vi "Configuration Utility.vi"() -> ()   [LabVIEW 2014, in "Standard Editor.lvlib"]
doc: "This is the main VI for the configuration editor."
uses:
  Standard Editor.lvlib
  Controls/StateCluster.ctl
  Configuration Editor/Classes/SystemConfigRepo/SystemConfigRepo.lvclass
  Configuration Editor/Classes/Systems/Systems.lvclass
  <vilib>/NI/Configuration Framework/Node/StandardEvents.ctl
  <vilib>/NI/Configuration Framework/Node/UserEventRef.ctl
  <vilib>/NI/Configuration Framework/Controls/EventCluster.ctl
  <vilib>/NI/Configuration Framework/Node/NodeChangeEvent.ctl
  <vilib>/NI/Configuration Framework/Node/NodeRef.ctl
  <vilib>/NI/Configuration Framework/Node/NISE_CEF_Node.lvclass
  <vilib>/NI/Configuration Framework/Node/CacheState.ctl
  <vilib>/NI/Configuration Framework/Node/RefreshUIEvent.ctl
  <vilib>/NI/Configuration Framework/Node/StopEvent.ctl
  <vilib>/NI/Configuration Framework/glyph manager/glyph manager.ctl
  <vilib>/picture/picture.llb/imagedata.ctl
  <vilib>/NI/AMC/Message Queue.ctl
  <vilib>/NI/AMC/Message.ctl
  <vilib>/NI/Tools/Keyed Array/KeyedArray.ctl
  Controls/add message.ctl
  Controls/MoveMessage.ctl
  <vilib>/NI/Progress Bar/Controls/Progress Bar Properties.ctl
  <vilib>/NI/Progress Bar/Controls/Update Bar Actions.ctl
  <vilib>/NI/AMC/Create Single Message.vi
  <vilib>/NI/AMC/Update Message Routing Info.vi
  <vilib>/NI/AMC/Read Termination Message.vi
  Configuration Editor/subVIs/Glyphs Status.ctl
  Configuration Editor/subVIs/Add status to name.vi
  <vilib>/NI/AMC/Send Message.vi
  <vilib>/NI/AMC/Globals.vi
  Configuration Editor/Classes/Module editor node/module editor node.lvclass
  Configuration Editor/Classes/EngineTags/EngineTags.lvclass
  <vilib>/NI/Module Timing Source/timing source/TBM timing source.lvclass
  Configuration Editor/Classes/TBM Configuration Node/TBM Configuration Node.lvclass
  <vilib>/NI/Tag Bus Module Framework/root configuration/TBM configuration.lvclass
  Framework Configuration Classes/target configuration/PL_Target Configuration.lvclass
  Configuration Editor/Classes/Targets/Targets.lvclass
  Configuration Editor/Classes/Engine Parent/Engine Parent Editor Node.lvclass
  <vilib>/NI/Configuration Framework/Repository/NISE_CEF_Repository.lvclass
  Framework Configuration Classes/system configuration/PL_System Configuration.lvclass
  <vilib>/NI/Module Execution Interface/Engine Configuration/engine configuration.lvclass
  <vilib>/NI/Tag Bus Module Framework/channel/TBM channel.lvclass
  <vilib>/NI/Tag Bus Module Framework/module configuration/TBM module configuration.lvclass
  <vilib>/NI/AMC/AMC.lvlib
  <vilib>/NI/Configuration Framework/NISE_CEF_TreeControl.lvlib
  Framework Configuration Classes/class cache/PL_class cache.lvlib
  Configuration Editor/PL Framework Configuration Tool.lvlib
  <vilib>/NI/Configuration Framework/hierarchy repo/NISE_CEF_HierarchyRepo.lvclass
  <vilib>/NI/Configuration Framework/tree serializer/NISE_CEF_TreeSerializer.lvlib
  <vilib>/NI/Configuration Framework/glyph manager/glyph manager.lvlib
  <vilib>/NI/Tools/Keyed Array/Tools_KeyedArray.lvlib
  <vilib>/NI/Progress Bar/Progress Bar.lvlib
  about menu/About Screen Library.lvlib
  INI Configuration/DCAF INI.lvlib
panel:
  in  "Exit":bool
  in  "View":string(tree)
  # "DCAF Editor"
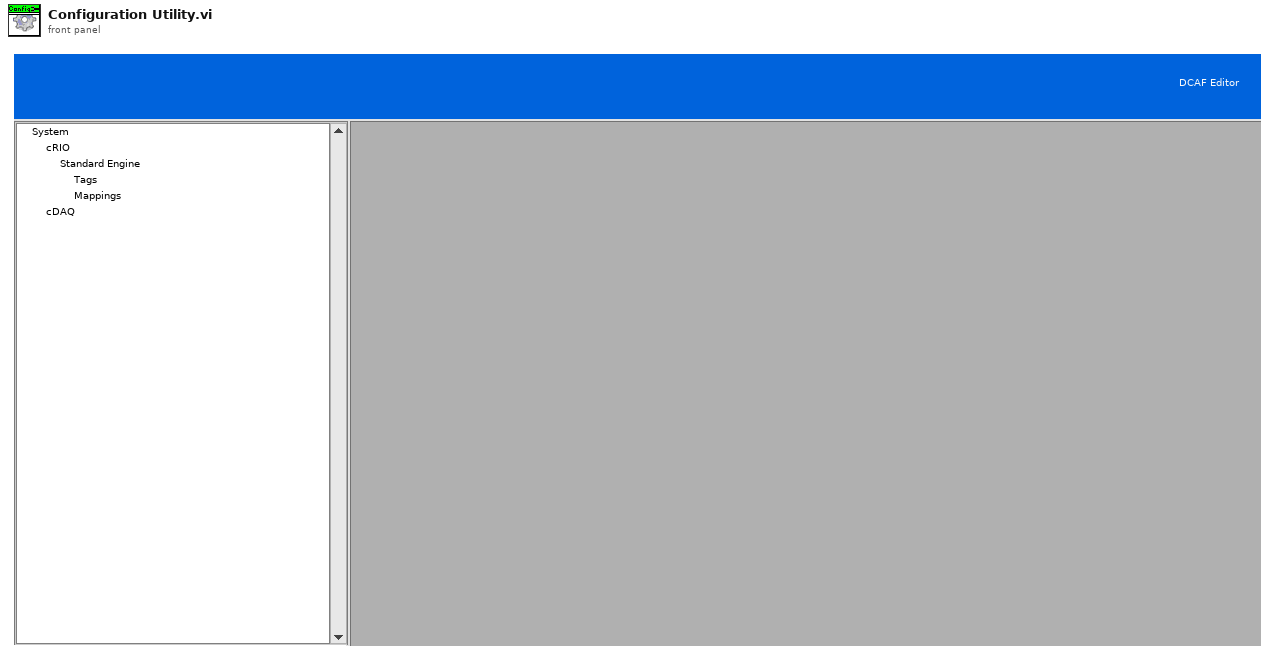
[diagram p1: front panel]
types:
  T1 = enum32{"Invalid", "Standard", "Closed", "Hidden", "Minimized", "Maximized"}
  T2 = typedef "Standard Editor.lvlib/StateCluster.ctl" = cluster{"repository":refnum<class "SystemConfigRepo.lvclass">, "root":refnum<data-value>, "unsaved changes":bool, "current path":path, "classes cache":path, "standard events":T3, "glyph manager":T9, "VI ref":refnum<vi>, "main queue":T11, "Sub Panel":refnum<vi>}
  T3 = typedef "NISE_CEF_Node.lvclass/StandardEvents.ctl" = cluster{"user event":T4, "node change":T5, "cache state":T6, "refresh UI":T7, "stop event":T8}
  T4 = typedef "NISE_CEF_Node.lvclass/UserEventRef.ctl" = refnum<user-event>
  T5 = typedef "NISE_CEF_Node.lvclass/NodeChangeEvent.ctl" = refnum<user-event>
  T6 = typedef "NISE_CEF_Node.lvclass/CacheState.ctl" = refnum<user-event>
  T7 = typedef "NISE_CEF_Node.lvclass/RefreshUIEvent.ctl" = refnum<user-event>
  T8 = typedef "NISE_CEF_Node.lvclass/StopEvent.ctl" = refnum<user-event>
  T9 = typedef "glyph manager.lvlib/glyph manager.ctl" = cluster{"search paths":path[], "glyph map":variant, "base glyphs":T10[], "desired overlays":string[]}
  T10 = typedef "imagedata.ctl" = cluster{"image type":i32, "image depth":i32, "image":u8[], "mask":u8[], "colors":u32[], "Rectangle":cluster{"left":i16, "top":i16, "right":i16, "bottom":i16}}
  T11 = typedef "AMC.lvlib/Message Queue.ctl" = refnum<queue>
  T12 = cluster{"node id":string, "RightClickPath":string}
  T13 = typedef "Standard Editor.lvlib/add message.ctl" = cluster{"node type":string, "to add to":string}
  T14 = typedef "Standard Editor.lvlib/MoveMessage.ctl" = cluster{"node ref":T15, "new parent":T15, "Index":i32}
  T15 = typedef "NISE_CEF_Node.lvclass/NodeRef.ctl" = refnum<data-value>
  T16 = typedef "LVPoint32TypeDef.ctl" = cluster{"Horizontal":i32, "Vertical":i32}
  T17 = cluster{"data name":string, "drag data":variant}[]
  T18 = typedef "NISE_CEF_Node.lvclass/NodeMenuOptions.ctl" = cluster{"removable":bool, "movable":bool, "duplicate":bool}
  T19 = typedef "Progress Bar.lvlib/Progress Bar Properties.ctl" = cluster{"Background Color":u32, "Installer Title":string, "Title Color":u32, "Action Text":string, "Text Color":u32, "Slider Value":u8, "Bar Color":u32, "Timeout":i32}
  T20 = typedef "Progress Bar.lvlib/Update Bar Actions.ctl" = enum16{"Add To Existing", "Set to Value"}
  T21 = typedef "Standard Editor.lvlib/FilePaths.ctl" = cluster{"glyphs":path[], "classes":path, "classes cache":path}
  T22 = typedef "PL_class cache.lvlib/cache definition.ctl" = cluster{"configuration":T23, "class cache data":T24}
  T23 = typedef "PL_class cache.lvlib/cache search configuration.ctl" = cluster{"Search Paths":path[], "Folders to Exclude":string[], "full class list":path[]}
  T24 = typedef "PL_class cache.lvlib/cached class information.ctl" = cluster{"targets":T25[], "engines":T26[], "modules":T26[], "ignored class list":path[]}
  T25 = typedef "PL_class cache.lvlib/target class metadata.ctl" = cluster{"file name":string, "fully qualified name":string, "menu display name":string, "configuration class name":string}
  T26 = typedef "PL_class cache.lvlib/class metadata.ctl" = cluster{"file name":string, "fully qualified name":string, "menu display name":string, "configuration class":string, "category":string, "instances allowed":i32, "supported targets":T27[]}
  T27 = typedef "TBM configuration.lvclass/Target Types.ctl" = enum16{"Windows", "Mac", "Linux", "Linux RT ARM", "VxWorks", "Pharlap", "Other", "Linux RT x64"}
  T28 = typedef "NISE_CEF_Node.lvclass/Summary.ctl" = cluster{"ID":string, "parent ID":string, "node type":string, "text":string, "additional text":string, "glyph":string, "depth":i32, "glyph overlay":string}
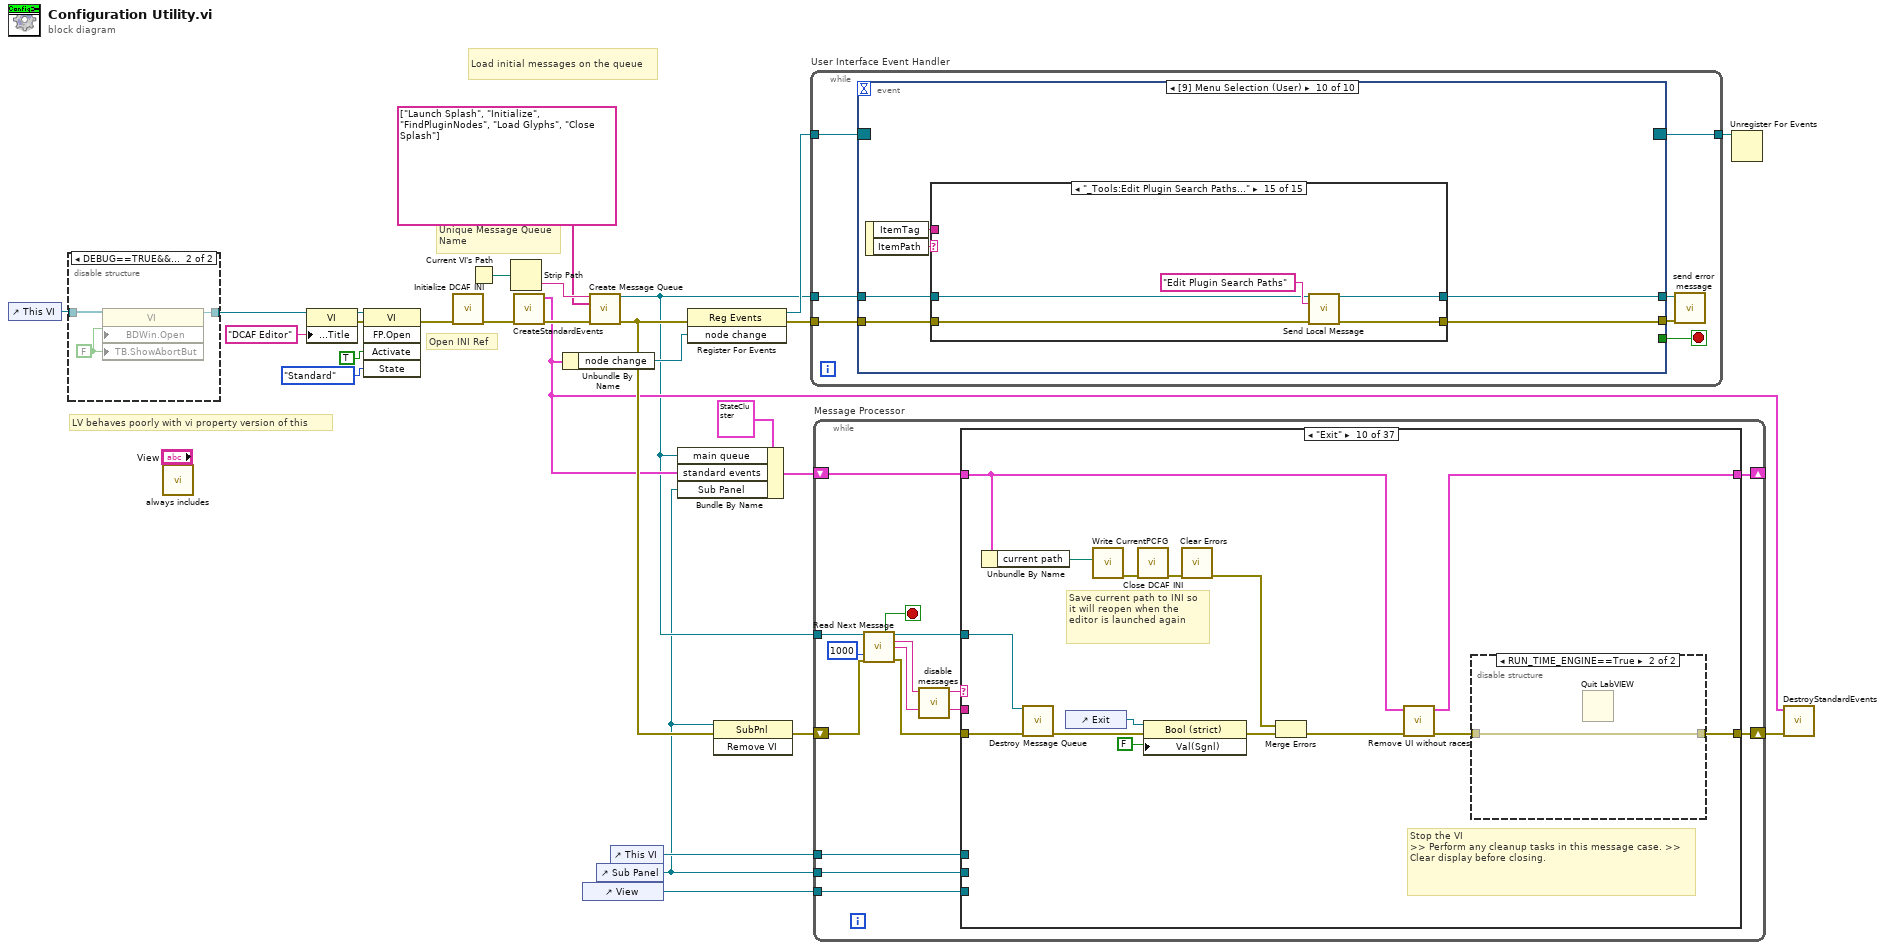
[diagram p0: block diagram]
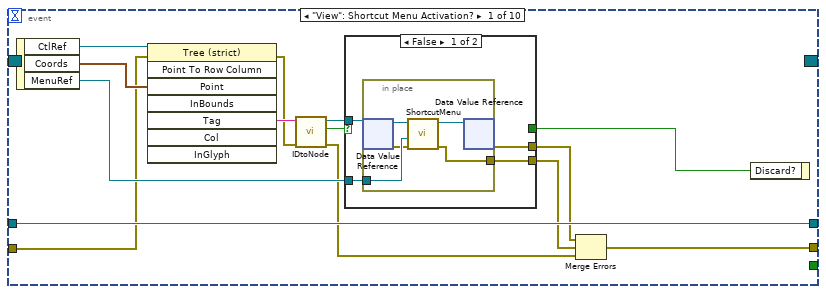
[diagram p3: hidden frame]
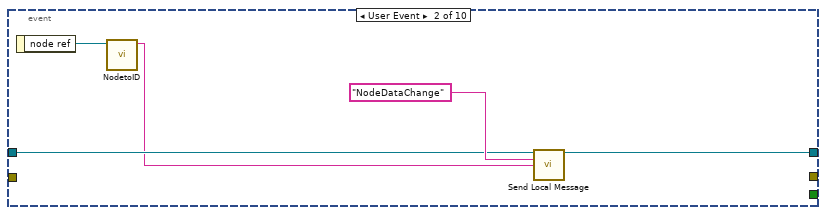
[diagram p5: hidden frame]
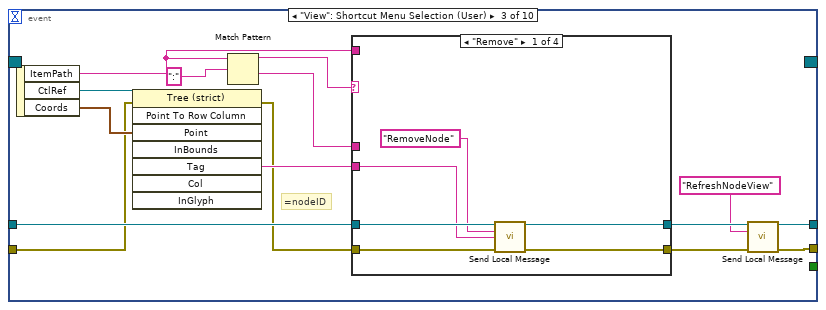
[diagram p6: hidden frame]
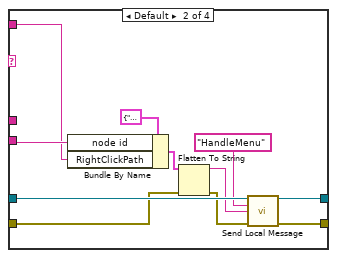
[diagram p7: hidden frame]
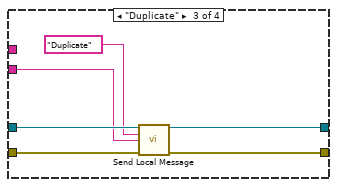
[diagram p8: hidden frame]
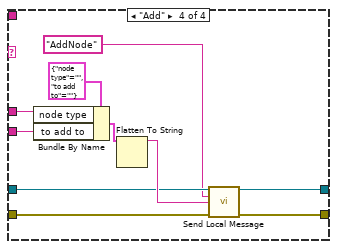
[diagram p9: hidden frame]
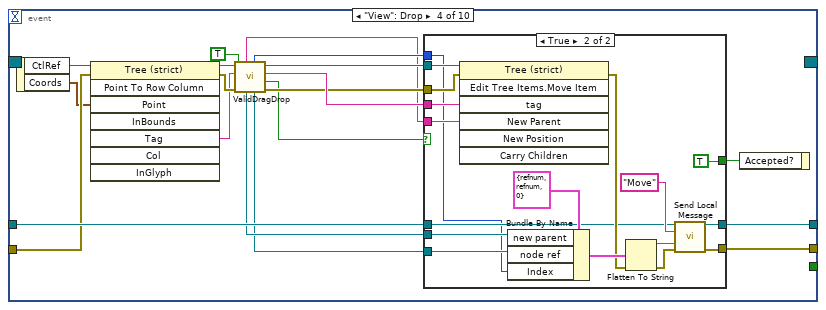
[diagram p10: hidden frame]
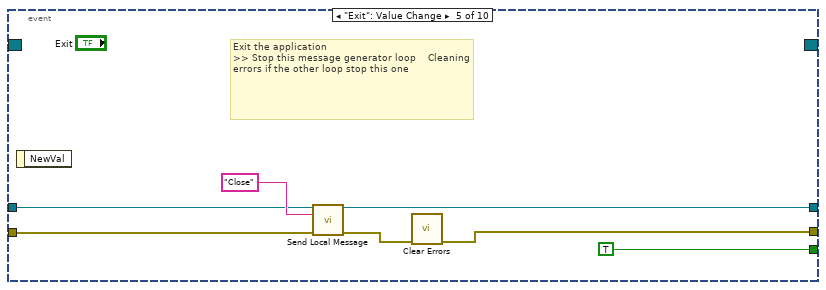
[diagram p12: hidden frame]
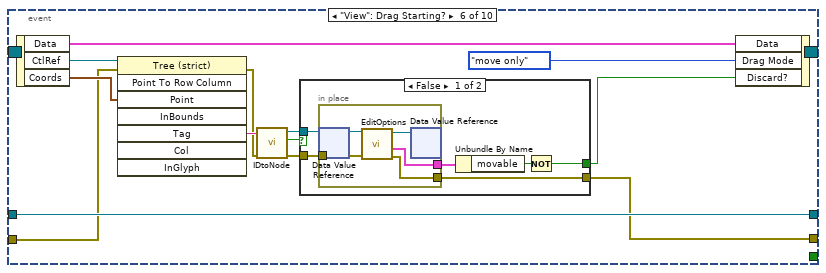
[diagram p13: hidden frame]
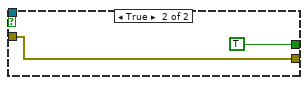
[diagram p14: hidden frame]
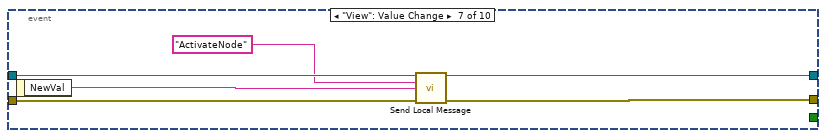
[diagram p15: hidden frame]
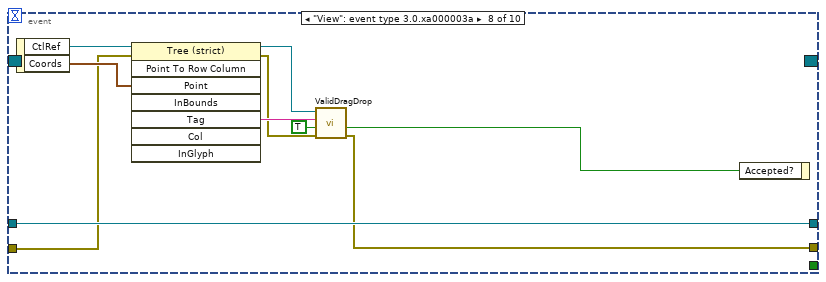
[diagram p16: hidden frame]
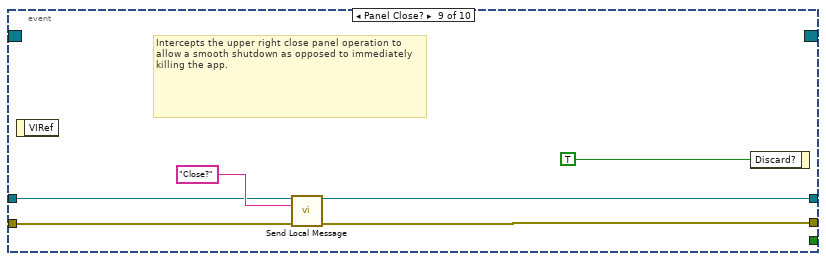
[diagram p17: hidden frame]
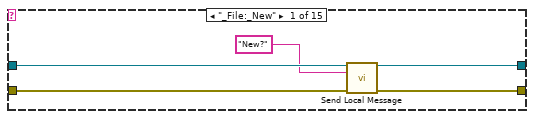
[diagram p18: hidden frame]
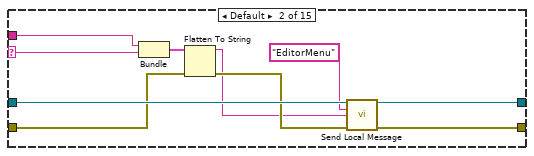
[diagram p19: hidden frame]
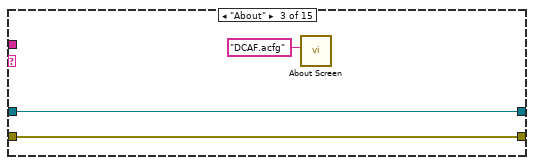
[diagram p20: hidden frame]
diagram:
  # "Open INI Ref"
  # "LV behaves poorly with vi property version of this"
  # "Unique Message Queue Name"
  # "Load initial messages on the queue"
  n1 = control-ref of="This VI"() -> (w20:refnum<vi>)
  n2 = disable-structure shown="DEBUG==TRUE&&RUN_TIME_ENGINE==False" {
    disable-tunnel: [w28 w31] -> w5
    disable-tunnel: w20 -> [w28 w30]
    frame condition #0 (active) {
    }
    frame condition #1 {
      w29 = FALSE ("Block Diagram Window:Open")
      n3 = property class="VI"(reference=w30, "BDWin.Open"=w29, "TB.ShowAbortBut"=w29) -> (reference out=w31:refnum<vi>)  [unwired: 1 in, 1 out]
    }
  }
  n4 = call "always includes.vi"() -> ()  [unwired: 12 in]
  n5 = property class="VI"(reference=w5, "Front Panel.Title"="DCAF Editor" ("Front Panel Window:Title")) -> (reference out=w4:refnum<vi>, error out=w6:errorcluster)  [unwired: 1 in]
  n6 = invoke class="VI" method="FP.Open"(reference=w4, error in=w6, "Activate"=TRUE ("Activate?"), "State"=T1."Standard") -> (error out=w1:errorcluster)  [unwired: 1 in, 4 out]
  n7 = call "Initialize DCAF INI.vi"("Error In"=w1) -> ("Error Out"=w2:errorcluster)  [unwired: 10 in]
  n8 = Current VI's Path() -> (path=w26:path)
  n9 = Strip Path(path=w26) -> (name=w27:string)  [unwired: 1 out]
  n10 = call <vilib>:"CreateStandardEvents.vi"("error in"=w2) -> ("error out"=w16:errorcluster, "standard events"=w9:T3)  [unwired: 9 in]
  n11 = Unbundle By Name(w9) -> ("node change"=w14:T5)
  n12 = control-ref of="View"() -> (w19:refnum<vi>)
  n13 = call <vilib>:"Create Message Queue.vi"("message queue name"=w27, "initial message names"=string[] ["Launch Splash", "Initialize", "FindPluginNodes", "Load Glyphs", "Close Splash"], "error in"=w16) -> ("message queue out"=w8:T11, "error out"=w23:errorcluster)  [unwired: 11 in]
  n14 = control-ref of="Sub Panel"() -> (w7:refnum<vi>)
  n15 = control-ref of="This VI"() -> (w17:refnum<vi>)
  n16 = Bundle By Name(cluster=T2 {"repository"=refnum, "root"=refnum, "unsaved changes"=FALSE, "current path"=path "", "classes cache"=path "", "standard events"={"user event"=refnum, "node change"=refnum, "cache state"=refnum, "refresh UI"=refnum, "stop event"=refnum}, "glyph manager"={"search paths"=[], "glyph map"=variant, "base glyphs"=[], "desired overlays"=[]}, "VI ref"=refnum, "main queue"=refnum, "Sub Panel"=refnum}, "main queue"=w8, "standard events"=w9, "Sub Panel"=w7) -> (w12:T2)
  n17 = register-events(error in=w23, w14) -> (reference out=w13:refnum<event-registration>, error out=w15:errorcluster)  [unwired: 1 in]
  n18 = invoke class="SubPnl" method="Remove VI"(reference=w7, error in=w23) -> (error out=w18:errorcluster)  [unwired: 1 in, 2 out]
  n19 = while "User Interface Event Handler" {
    tunnel: w8 -> [w38]
    tunnel: w15 -> [w34]
    tunnel: w13 -> [w33]
    tunnel: [w32] -> w11
    stop <- w37 stop-if-true
    n20 = event shown="[9] Menu Selection (User)" {
      selector: w33 -> [_ _ _ _ _ _ _ _ _ _]
      dyn-events: [_ _ _ _ _ _ _ _ _ _] -> w32
      timeout: _ -> [_ _ _ _ _ _ _ _ _ _]
      tunnel: w38 -> [w46 w65 w77 w125 w158 w165 w192 w197 w207 w213]
      tunnel: [_ _ _ _ TRUE _ _ _ _ _] -> w37
      tunnel: [w46 w64 w69 w127 w154 w165 w189 w197 w205 w212] -> w36
      tunnel: [w41 _ w70 w126 w155 w161 w188 w194 w203 w210] -> w35
      tunnel: w34 -> [w45 _ w75 w124 w156 w164 w187 w196 w204 w211]
      event "View": Shortcut Menu Activation? {
        n21 = event-data() -> ("CtlRef"=w52:refnum<vi>, "Coords"=w51:T16, "MenuRef"=w48:refnum<k9>)  [unwired: 1 in]
        n22 = invoke class="Tree (strict)" method="Point To Row Column"(reference=w52, error in=w45, "Point"=w51) -> (error out=w44:errorcluster, "Tag"=w50:string)  [unwired: 5 in, 6 out]
        n23 = call <vilib>:"IDtoNode.vi"("error in"=w44, "ID"=w50) -> ("error out"=w42:errorcluster, "invalid Id"=w47:bool, "node ref"=w49:T15)  [unwired: 7 in]
        n24 = case shown="False" w47 {
          selector: w47 -> [_ w62]
          tunnel: w49 -> [w56 _]
          tunnel: w48 -> [w55 _]
          tunnel: [w54 _] -> w43
          tunnel: [w53 _] -> w40
          tunnel: [_ w62] -> w39
          frame False {
            n25 = in-place {
              in-place-border: w55 -> [w59]
              in-place-border: [w57] -> w54
              n26 = in-place-dvr #1(w56) -> (w61:refnum<class "NISE_CEF_Node.lvclass">, w58:errorcluster)
              n27 = call-dynamic "ShortcutMenu.vi"("error in"=w58, "menu ref in"=w59, "node in"=w61) -> ("error out"=w57:errorcluster, "node out"=w60:refnum<class "NISE_CEF_Node.lvclass">)  [unwired: 6 in, 1 out]
              n28 = in-place-dvr #1(w60) -> (w53:errorcluster)  [unwired: 1 out]
            }
          }
          frame True {
          }
        }
        n29 = Merge Errors(w40, w43, w42) -> (w41:errorcluster)
        n30 = event-data("Discard?"=w39) -> ()  [unwired: 1 in, 1 out]
      }
      event User Event {
        n31 = event-data() -> ("node ref"=w67:T15)  [unwired: 1 in]
        n32 = call <vilib>:"NodetoID.vi"("node ref"=w67) -> ("ID"=w63:string)  [unwired: 9 in, 1 out]
        n33 = call <vilib>:"Send Local Message.vi"("message queue in"=w65, "message name"="NodeDataChange", "message value"=w63) -> ("message queue out"=w64:T11)  [unwired: 10 in, 2 out]
      }
      event "View": Shortcut Menu Selection (User) {
        # "=nodeID"
        n34 = event-data() -> ("ItemPath"=w73:string, "CtlRef"=w80:refnum<vi>, "Coords"=w81:T16)  [unwired: 1 in]
        n35 = invoke class="Tree (strict)" method="Point To Row Column"(reference=w80, error in=w75, "Point"=w81) -> (error out=w74:errorcluster, "Tag"=w76:string)  [unwired: 5 in, 6 out]
        n36 = Match Pattern(string=w73, regular expression=":") -> (before substring=w79:string, after substring=w78:string)  [unwired: 1 in, 2 out]
        n37 = case shown="\"Remove\"" w79 {
          tunnel: w78 -> [_ _ _ w110]
          tunnel: w77 -> [w88 w99 w105 w112]
          tunnel: w76 -> [w86 w93 w103 w111]
          tunnel: [w85 w97 w102 w108] -> w72
          tunnel: [w84 w96 w100 w106] -> w71
          tunnel: w74 -> [w83 w92 w101 w107]
          tunnel: w73 -> [_ w89 _ _]
          frame "Remove" {
            n38 = call <vilib>:"Send Local Message.vi"("message queue in"=w88, "message name"="RemoveNode" ("Message Name"), "message value"=w86, "error in"=w83) -> ("message queue out"=w85:T11, "error out"=w84:errorcluster)  [unwired: 9 in, 1 out]
          }
          frame Default {
            n39 = Bundle By Name(cluster=T12 {"node id"="", "RightClickPath"=""} ("input cluster"), "node id"=w93, "RightClickPath"=w89) -> (w94:T12)
            n40 = Flatten To String(anything=w94, error in (no error)=w92) -> (data string=w90:string, error out=w91:errorcluster)  [unwired: 2 in, 1 out]
            n41 = call <vilib>:"Send Local Message.vi"("message queue in"=w99, "message name"="HandleMenu" ("Message Name"), "message value"=w90, "error in"=w91) -> ("message queue out"=w97:T11, "error out"=w96:errorcluster)  [unwired: 9 in, 1 out]
          }
          frame "Duplicate" {
            n42 = call <vilib>:"Send Local Message.vi"("message queue in"=w105, "message name"="Duplicate" ("Message Name"), "message value"=w103, "error in"=w101) -> ("message queue out"=w102:T11, "error out"=w100:errorcluster)  [unwired: 9 in, 1 out]
          }
          frame "Add" {
            n43 = Bundle By Name(cluster=T13 {"node type"="", "to add to"=""} ("input cluster"), "node type"=w110, "to add to"=w111) -> (w113:T13)
            n44 = Flatten To String(anything=w113) -> (data string=w114:string)  [unwired: 3 in, 2 out]
            n45 = call <vilib>:"Send Local Message.vi"("message queue in"=w112, "message name"="AddNode" ("Message Name"), "message value"=w114, "error in"=w107) -> ("message queue out"=w108:T11, "error out"=w106:errorcluster)  [unwired: 9 in, 1 out]
          }
        }
        n46 = call <vilib>:"Send Local Message.vi"("message queue in"=w72, "message name"="RefreshNodeView", "error in"=w71) -> ("message queue out"=w69:T11, "error out"=w70:errorcluster)  [unwired: 10 in, 1 out]
      }
      event "View": Drop {
        n47 = event-data() -> ("CtlRef"=w123:refnum<vi>, "Coords"=w122:T16)  [unwired: 1 in]
        n48 = invoke class="Tree (strict)" method="Point To Row Column"(reference=w123, error in=w124, "Point"=w122) -> (reference out=w133:refnum<vi>, error out=w132:errorcluster, "Tag"=w130:string)  [unwired: 5 in, 5 out]
        n49 = call <vilib>:"ValidDragDrop.vi"("error in"=w132, "Reorder"=TRUE, "drag over"=w130, "Tree Ref in"=w133) -> ("Error Out"=w129:errorcluster, "Accepted"=w116:bool, "Drag"=w131:string, "Tree Ref out"=w134:refnum<vi>, "Moved Node"=w120:T15, "Position"=w119:i32, "Parent Node"=w121:T15, "Parent"=w118:string)
        n50 = case shown="True" w116 {
          tunnel: w131 -> [_ w151]
          tunnel: w134 -> [_ w153]
          tunnel: [_ TRUE] -> w128
          tunnel: w118 -> [_ w149]
          tunnel: w125 -> [w136 w138]
          tunnel: [w136 w145] -> w127
          tunnel: [w135 w144] -> w126
          tunnel: w120 -> [_ w140]
          tunnel: w121 -> [_ w139]
          tunnel: w129 -> [w135 w141]
          tunnel: w119 -> [_ w137]
          frame False {
          }
          frame True {
            n51 = invoke class="Tree (strict)" method="Edit Tree Items.Move Item"(reference=w153, error in=w141, "tag"=w151, "New Parent"=w149) -> (error out=w142:errorcluster)  [unwired: 3 in, 6 out]
            n52 = Bundle By Name(cluster=T14 {"node ref"=refnum, "new parent"=refnum, "Index"=0} ("Cluster"), "new parent"=w139, "node ref"=w140, "Index"=w137) -> (w148:T14)
            n53 = Flatten To String(anything=w148, error in (no error)=w142) -> (data string=w147:string, error out=w143:errorcluster)  [unwired: 2 in, 1 out]
            n54 = call <vilib>:"Send Local Message.vi"("message queue in"=w138, "message name"="Move", "message value"=w147, "error in"=w143) -> ("message queue out"=w145:T11, "error out"=w144:errorcluster)  [unwired: 9 in, 1 out]
          }
        }
        n55 = event-data("Accepted?"=w128) -> ()  [unwired: 1 in, 1 out]
      }
      event "Exit": Value Change {
        # "Exit the application                                           >> Stop this message generator loop    Cleaning errors if the other loop stop this one"
        n56 = event-data() -> ()  [unwired: 1 in, 1 out]
        n57 = call <vilib>:"Send Local Message.vi"("message queue in"=w158, "message name"="Close", "error in"=w156) -> ("message queue out"=w154:T11, "error out"=w159:errorcluster)  [unwired: 10 in, 1 out]
        n58 = call <vilib>:"Clear Errors.vi"("error in (no error)"=w159) -> ("error out"=w155:errorcluster)  [unwired: 5 in, 1 out]
      }
      event "View": Drag Starting? {
        n59 = event-data() -> ("Data"=w171:T17, "CtlRef"=w173:refnum<vi>, "Coords"=w172:T16)  [unwired: 1 in]
        n60 = invoke class="Tree (strict)" method="Point To Row Column"(reference=w173, error in=w164, "Point"=w172) -> (error out=w163:errorcluster, "Tag"=w170:string)  [unwired: 5 in, 6 out]
        n61 = call <vilib>:"IDtoNode.vi"("error in"=w163, "ID"=w170) -> ("error out"=w162:errorcluster, "invalid Id"=w169:bool, "node ref"=w168:T15)  [unwired: 7 in]
        n62 = case shown="False" w169 {
          tunnel: w168 -> [w179 _]
          tunnel: [w176 TRUE ("Removable")] -> w166
          tunnel: w162 -> [w175 w185]
          tunnel: [w174 w185] -> w161
          frame False {
            n63 = in-place {
              in-place-border: [w182] -> w178
              in-place-border: w175 -> [w181]
              in-place-border: [w180] -> w174
              n64 = in-place-dvr #2(w179) -> (w184:refnum<class "NISE_CEF_Node.lvclass">)  [unwired: 1 out]
              n65 = call-dynamic "EditOptions.vi"("error in"=w181, "node in"=w184) -> ("error out"=w180:errorcluster, "edit options"=w182:T18, "node out"=w183:refnum<class "NISE_CEF_Node.lvclass">)  [unwired: 6 in, 1 out]
              n66 = in-place-dvr #2(w183) -> ()  [unwired: 2 out]
            }
            n67 = Unbundle By Name(w178) -> ("movable"=w177:bool)
            n68 = Not(x=w177) -> (.not. x?=w176:bool)
          }
          frame True {
          }
        }
        n69 = event-data("Data"=w171, "Drag Mode"=enum32{"copy or move", "copy only", "move only"}."move only", "Discard?"=w166) -> ()  [unwired: 1 in, 1 out]
      }
      event "View": Value Change {
        n70 = event-data() -> ("NewVal"=w190:string)  [unwired: 1 in]
        n71 = call <vilib>:"Send Local Message.vi"("message queue in"=w192, "message name"="ActivateNode" ("Message Name"), "message value"=w190, "error in"=w187) -> ("message queue out"=w189:T11, "error out"=w188:errorcluster)  [unwired: 9 in, 1 out]
      }
      event "View": event type 3.0.xa000003a {
        n72 = event-data() -> ("CtlRef"=w202:refnum<vi>, "Coords"=w199:T16)  [unwired: 1 in]
        n73 = invoke class="Tree (strict)" method="Point To Row Column"(reference=w202, error in=w196, "Point"=w199) -> (reference out=w201:refnum<vi>, error out=w195:errorcluster, "Tag"=w200:string)  [unwired: 5 in, 5 out]
        n74 = call <vilib>:"ValidDragDrop.vi"("error in"=w195, "Reorder"=TRUE, "drag over"=w200, "Tree Ref in"=w201) -> ("Error Out"=w194:errorcluster, "Accepted"=w198:bool)  [unwired: 6 out]
        n75 = event-data("Accepted?"=w198) -> ()  [unwired: 1 in, 1 out]
      }
      event Panel Close? {
        # "Intercepts the upper right close panel operation to allow a smooth shutdown as opposed to immediately killing the app."
        n76 = event-data() -> ()  [unwired: 1 in, 1 out]
        n77 = call <vilib>:"Send Local Message.vi"("message queue in"=w207, "message name"="Close?", "error in"=w204) -> ("message queue out"=w205:T11, "error out"=w203:errorcluster)  [unwired: 10 in, 1 out]
        n78 = event-data("Discard?"=TRUE) -> ()  [unwired: 1 in, 1 out]
      }
      event Menu Selection (User) {
        n79 = event-data() -> ("ItemTag"=w209:string, "ItemPath"=w214:string)  [unwired: 1 in]
        n80 = case shown="\"_Tools:Edit Plugin Search Paths...\"" w214 {
          selector: w214 -> [_ w225 _ _ _ _ _ _ _ _ _ _ _ _ _]
          tunnel: w213 -> [w219 w229 w232 w237 w242 w247 w252 w261 w266 w271 w276 w281 w286 w292 w296]
          tunnel: [w215 w226 w232 w233 w238 w243 w248 w258 w263 w268 w273 w278 w283 w289 w295] -> w212
          tunnel: w211 -> [w217 w228 w231 w235 w240 w245 w250 w257 w264 w269 w274 w279 w284 w290 w294]
          tunnel: [w216 w227 w231 w234 w239 w244 w249 w255 w262 w267 w272 w277 w282 w288 w293] -> w210
          tunnel: w209 -> [_ w224 _ _ _ _ _ _ _ _ _ _ _ _ _]
          frame "_File:_New" {
            n81 = call <vilib>:"Send Local Message.vi"("message queue in"=w219, "message name"="New?" ("Message Name"), "error in"=w217) -> ("message queue out"=w215:T11, "error out"=w216:errorcluster)  [unwired: 10 in, 1 out]
          }
          frame Default {
            n82 = Bundle("ItemTag"=w224, w225) -> (w221:cluster{"ItemTag":string, string})  [unwired: 1 in]
            n83 = Flatten To String(anything=w221, error in (no error)=w228) -> (data string=w220:string, error out=w222:errorcluster)  [unwired: 2 in, 1 out]
            n84 = call <vilib>:"Send Local Message.vi"("message queue in"=w229, "message name"="EditorMenu" ("Message Name"), "message value"=w220, "error in"=w222) -> ("message queue out"=w226:T11, "error out"=w227:errorcluster)  [unwired: 9 in, 1 out]
          }
          frame "About" {
            n85 = call "About Screen.vi"("About Config File Name"="DCAF.acfg") -> ()  [unwired: 11 in]
          }
          frame "_File:_Open..." {
            n86 = call <vilib>:"Send Local Message.vi"("message queue in"=w237, "message name"="Open?" ("Message Name"), "error in"=w235) -> ("message queue out"=w233:T11, "error out"=w234:errorcluster)  [unwired: 10 in, 1 out]
          }
          frame "_File:_Save" {
            n87 = call <vilib>:"Send Local Message.vi"("message queue in"=w242, "message name"="Save" ("Message Name"), "error in"=w240) -> ("message queue out"=w238:T11, "error out"=w239:errorcluster)  [unwired: 10 in, 1 out]
          }
          frame "_File:Save As..." {
            n88 = call <vilib>:"Send Local Message.vi"("message queue in"=w247, "message name"="SaveAs" ("Message Name"), "error in"=w245) -> ("message queue out"=w243:T11, "error out"=w244:errorcluster)  [unwired: 10 in, 1 out]
          }
          frame "_File:_Exit" {
            n89 = call <vilib>:"Send Local Message.vi"("message queue in"=w252, "message name"="Close?" ("Message Name"), "error in"=w250) -> ("message queue out"=w248:T11, "error out"=w249:errorcluster)  [unwired: 10 in, 1 out]
          }
          frame "_Tools:Multiple Parameter Editor" {
            n90 = call <vilib>:"Send Local Message.vi"("message queue in"=w261, "message name"="CleansubPanel", "error in"=w257) -> ("message queue out"=w260:T11, "error out"=w256:errorcluster)  [unwired: 10 in, 1 out]
            n91 = call <vilib>:"Send Local Message.vi"("message queue in"=w260, "message name"="Custom View", "message value"="Multiple Parameter Editor" ("Message Name"), "error in"=w256) -> ("message queue out"=w258:T11, "error out"=w255:errorcluster)  [unwired: 9 in, 1 out]
          }
          frame "_Tools:Test" {
            n92 = call <vilib>:"Send Local Message.vi"("message queue in"=w266, "message name"="Test", "error in"=w264) -> ("message queue out"=w263:T11, "error out"=w262:errorcluster)  [unwired: 10 in, 1 out]
          }
          frame "_Tools:Deploy Tool..." {
            n93 = call <vilib>:"Send Local Message.vi"("message queue in"=w271, "message name"="DeployTool?", "error in"=w269) -> ("message queue out"=w268:T11, "error out"=w267:errorcluster)  [unwired: 10 in, 1 out]
          }
          frame "_Tools:Save Binary..." {
            n94 = call <vilib>:"Send Local Message.vi"("message queue in"=w276, "message name"="Save Binary", "error in"=w274) -> ("message queue out"=w273:T11, "error out"=w272:errorcluster)  [unwired: 10 in, 1 out]
          }
          frame "_Tools:Script Include VI..." {
            n95 = call <vilib>:"Send Local Message.vi"("message queue in"=w281, "message name"="Script Include VI", "error in"=w279) -> ("message queue out"=w278:T11, "error out"=w277:errorcluster)  [unwired: 10 in, 1 out]
          }
          frame "_Tools:Load Binary..." {
            n96 = call <vilib>:"Send Local Message.vi"("message queue in"=w286, "message name"="Load Binary", "error in"=w284) -> ("message queue out"=w283:T11, "error out"=w282:errorcluster)  [unwired: 10 in, 1 out]
          }
          frame "_Tools:Refresh Plugins" {
            n97 = call <vilib>:"Send Local Message.vi"("message queue in"=w292, "message name"="FindPluginNodes", "message value"="Refresh", "error in"=w290) -> ("message queue out"=w289:T11, "error out"=w288:errorcluster)  [unwired: 9 in, 1 out]
          }
          frame "_Tools:Edit Plugin Search Paths..." {
            n98 = call <vilib>:"Send Local Message.vi"("message queue in"=w296, "message name"="Edit Plugin Search Paths", "error in"=w294) -> ("message queue out"=w295:T11, "error out"=w293:errorcluster)  [unwired: 10 in, 1 out]
          }
        }
      }
    }
    n99 = call "send error message.vi"("error in"=w35, "message queue in"=w36) -> ()  [unwired: 9 in, 1 out]
  }
  n100 = while "Message Processor" {
    shift-right: [w310] -> w10
    shift-left: w18 -> [w309]
    tunnel: w8 -> [w308]
    shift-right: [w306] -> _
    shift-left: w12 -> [w305]
    tunnel: w17 -> [w300]
    tunnel: w7 -> [w299]
    tunnel: w19 -> [w298]
    stop <- w312 stop-if-true
    n101 = call <vilib>:"Read Next Message.vi"("message queue in"=w308, "timeout (1 ms)"=1000, "error in"=w309) -> ("exit process?"=w312:bool, "message queue out"=w304:T11, "message name"=w301:string, "message value"=w303:string, "error out"=w311:errorcluster)  [unwired: 5 in, 3 out]
    n102 = call "disable messages.vi"("message to check"=w301) -> ("message out"=w302:string)  [unwired: 10 in]
    n103 = case shown="\"Exit\"" w302 {
      selector: w302 -> [_ w316 _ _ _ _ _ _ _ _ _ w443 _ _ _ w599 _ _ _ _ _ _ _ _ _ _ _ _ _ _ _ _ _ _ _ _ _]
      tunnel: w303 -> [_ _ _ _ _ _ _ _ w404 _ _ _ _ w515 _ _ _ w618 _ _ w716 _ w774 w816 _ _ w860 w874 w898 _ w929 _ _ w990 w1007 _ w1016]
      tunnel: w311 -> [w314 w319 w321 w331 w340 w361 w385 w395 w405 w438 w442 w453 w500 w520 w554 w597 w609 w623 w643 w661 w691 w737 w775 w817 w825 w828 w838 w873 w899 w915 w928 w971 w980 w989 w1006 w1013 w1019]
      tunnel: [w314 w319 w321 w323 w335 w371 w388 w398 errorcluster {"status"=FALSE, "code"=0, "source"=""} ("error out") w436 w442 w456 w514 w517 w551 w601 w614 w622 w642 w649 w696 w736 w764 w804 w824 w828 w839 w863 w901 w915 w927 w968 w979 w988 w1005 w1011 w1018] -> w310
      tunnel: [w313 w315 w320 w325 w346 w370 w386 w396 w399 w430 w441 w444 w512 w521 w555 w602 w615 w619 w644 w662 w717 w733 w761 w812 w826 w827 w848 w868 w900 w916 w921 w964 w977 w982 w1001 w1012 w1015] -> w306
      tunnel: w305 -> [w313 w315 w320 w325 w349 w378 w386 w396 w400 w429 w441 w454 w499 w523 w560 w595 w608 w620 w644 w662 w717 w734 w762 w813 w826 w827 w831 w866 w894 w917 w919 w976 w978 w981 w1008 w1012 w1021]
      tunnel: w304 -> [_ _ _ _ w332 _ _ w397 w407 w437 _ w455 w513 w522 w559 w596 w613 w621 _ w646 _ w735 w766 w809 _ _ _ _ _ _ _ _ _ _ w1004 _ w1017]
      tunnel: w300 -> [_ _ _ w327 _ _ w387 _ _ _ _ _ _ _ _ _ _ _ _ _ _ _ _ _ _ _ _ _ _ _ _ w956 _ _ _ _ _]
      tunnel: w299 -> [_ _ _ _ _ _ _ _ _ _ _ _ _ _ _ _ _ _ _ _ _ _ _ _ _ _ _ _ _ _ w922 _ _ _ _ _ _]
      tunnel: w298 -> [_ _ _ _ _ w368 _ _ _ _ _ w448 _ _ _ _ _ _ _ _ _ _ w765 _ _ _ w849 w869 w895 _ w923 w970 _ _ _ _ _]
      frame "", "Idle" {
      }
      frame "Missing Message Handler", Default {
        # "Call this case if a message is received that is not handled by any other case. Typically this is a programming error as a result of a typo or unhandled message/missing message handler."
        n104 = Format Into String(format string="Internal Error: Missing message handler for '%s\" message." ("message"), w316) -> (resulting string=w318:string)  [unwired: 2 in, 1 out]
        n105 = One Button Dialog(message=w318) -> ()  [unwired: 2 out]
      }
      frame "------------Generic Operations------------" {
        # "Dummy case to add a seperation in the Case Structure menu"
      }
      frame "Launch Splash" {
        n106 = invoke class="VI" method="FP.Center"(reference=w327, error in=w331) -> (reference out=w330:refnum<vi>, error out=w329:errorcluster)  [unwired: 1 in, 1 out]
        n107 = invoke class="VI" method="FP.Open"(reference=w330, error in=w329, "State"=T1."Hidden") -> (error out=w326:errorcluster)  [unwired: 2 in, 4 out]
        n108 = call <vilib>:"Launch Progress Bar.vi"("error in (no error)"=w326) -> ("error out"=w324:errorcluster)  [unwired: 9 in, 1 out]
        n109 = call <vilib>:"Set All.vi"("error in (no error)"=w324, "Progress Bar Properties (Default)"=T19 {"Background Color"=3381759, "Installer Title"="Loading DCAF Editor", "Title Color"=0, "Action Text"="", "Text Color"=0, "Slider Value"=0, "Bar Color"=6618880, "Timeout"=10000}) -> ("error out"=w323:errorcluster)  [unwired: 9 in]
      }
      frame "Initialize" {
        # "issues in exe"
        n110 = Current VI's Menubar() -> (w339:refnum<k9>)
        n111 = call-dynamic "GenerateMenu.vi"("error in"=w340, "menu ref in"=w339, "SystemConfigRepo in"=refnum<class "SystemConfigRepo.lvclass"> refnum) -> ("error out"=w337:errorcluster)  [unwired: 6 in, 2 out]
        n112 = call "default file paths.vi"() -> ("paths"=w348:T21)  [unwired: 11 in]
        n113 = call <vilib>:"Set Action Text.vi"("error in (no error)"=w340, "Action Text"="Preparing UI...") -> ("error out"=w344:errorcluster)  [unwired: 9 in]
        n114 = Unbundle By Name(w348) -> ("classes cache"=w347:path)
        n115 = call <vilib>:"Update Progress Bar.vi"("Action"=Update_Bar_Actions."Set to Value", "error in (no error)"=w344, "Value"=u8 27) -> ("error out"=w343:errorcluster)  [unwired: 8 in]
        n116 = call <vilib>:"Clear Errors.vi"("error in (no error)"=w343) -> ()  [unwired: 5 in, 2 out]
        n117 = call "Read CurrentPCFG.vi"("Error In"=w337) -> ("Error Out"=w336:errorcluster, "Config File Exists?"=w334:bool, "Path Out"=w333:path)  [unwired: 8 in]
        n118 = Bundle By Name(cluster=w349, "classes cache"=w347) -> (w346:T2)
        n119 = case "Open Existing PCFG?" shown="True" w334 {
          tunnel: w336 -> [w353 w359]
          tunnel: [w352 w358] -> w335
          tunnel: w333 -> [_ w355]
          tunnel: w332 -> [w351 w357]
          frame False {
            n120 = call <vilib>:"Send Local Message.vi"("message queue in"=w351, "message name"="New", "error in"=w353) -> ("error out"=w352:errorcluster)  [unwired: 10 in, 2 out]
          }
          frame True {
            n121 = Path To String(path=w355) -> (string=w354:string)
            n122 = call <vilib>:"Send Local Message.vi"("message queue in"=w357, "message name"="Open", "message value"=w354, "error in"=w359) -> ("error out"=w358:errorcluster)  [unwired: 9 in, 2 out]
          }
        }
      }
      frame "Load Glyphs" {
        n123 = invoke class="Tree (strict)" method="Custom Item Symbols.Revert Symbols"(reference=w368, error in=w361) -> (reference out=w377:refnum<vi>, error out=w376:errorcluster)  [unwired: 1 in, 1 out]
        n124 = call <vilib>:"Set Action Text.vi"("error in (no error)"=w361, "Action Text"="Loading Glyphs...") -> ("error out"=w364:errorcluster)  [unwired: 9 in]
        n125 = call "default file paths.vi"() -> ("paths"=w367:T21)  [unwired: 11 in]
        n126 = call <vilib>:"Update Progress Bar.vi"("Action"=Update_Bar_Actions."Add To Existing", "error in (no error)"=w364, "Value"=u8 78) -> ("error out"=w360:errorcluster)  [unwired: 8 in]
        n127 = Unbundle By Name(w367) -> ("glyphs"=w366:path[])
        n128 = call <vilib>:"create glyph manager.vi"("error in"=w376, "tree ref (for default symbols)"=w377) -> ("error out"=w372:errorcluster, "glyph manager"=w373:T9)  [unwired: 8 in]
        n129 = call <vilib>:"Clear Errors.vi"("error in (no error)"=w360) -> ()  [unwired: 5 in, 2 out]
        n130 = for {
          tunnel: w366 -> [w379] mode=indexing
          shift-right: [w383] -> w375
          shift-left: w373 -> [w381]
          shift-right: [w382] -> w374
          shift-left: w372 -> [w380]
          n131 = call <vilib>:"add search path.vi"("error in"=w380, "search path"=w379, "glyph manager in"=w381) -> ("error out"=w382:errorcluster, "glyph manager out"=w383:T9)  [unwired: 7 in]
        }
        n132 = call <vilib>:"update tree control.vi"("error in"=w374, "tree reference"=w377, "glyph manager in"=w375) -> ("error out"=w371:errorcluster, "glyph manager out"=w369:T9)  [unwired: 7 in]
        n133 = Bundle By Name(cluster=w378, "glyph manager"=w369) -> (w370:T2)
      }
      frame "Close Splash" {
        n134 = call <vilib>:"Close Progress Bar.vi"("error in (no error)"=w385) -> ("error out"=w384:errorcluster)  [unwired: 9 in, 1 out]
        n135 = invoke class="VI" method="FP.Open"(reference=w387, error in=w384, "State"=T1."Standard") -> (reference out=w390:refnum<vi>, error out=w389:errorcluster)  [unwired: 2 in, 3 out]
        n136 = Close Reference(reference=w390, error in (no error)=w389) -> (error out=w388:errorcluster)
      }
      frame "Close" {
        n137 = Unbundle By Name(w396) -> ("root"=w393:refnum<data-value>)
        n138 = call <vilib>:"CloseNode.vi"("error in"=w395, "node ref"=w393) -> ("error out"=w392:errorcluster)  [unwired: 9 in]
        n139 = call <vilib>:"Send Local Message.vi"("message queue in"=w397, "message name"="Exit", "error in"=w392) -> ("error out"=w398:errorcluster)  [unwired: 10 in, 2 out]
      }
      frame "Error" {
        n140 = case shown="Default" w404 {
          selector: w404 -> [w409 _]
          tunnel: w405 -> [w410 w411]
          tunnel: [w408 w411] -> w402
          frame Default {
            n141 = Unflatten From String(type=w410, binary string=w409, error in (no error)=w410) -> (value=w408:errorcluster)  [unwired: 2 in, 2 out]
          }
          frame "" {
          }
        }
        n142 = call "Remove UI without races.vi"("error in"=w405, "state in"=w400) -> ("error out"=w401:errorcluster, "state out"=w399:T2)  [unwired: 8 in]
        n143 = call <vilib>:"Clear Errors.vi"("error in (no error)"=w401) -> ()  [unwired: 5 in, 2 out]
        n144 = Unbundle By Name(w402) -> ("code"=w403:i32)
        n145 = case shown="538500" w403 {
          tunnel: w407 -> [_ _ _ w417 _ _]
          tunnel: w402 -> [_ _ _ w416 w422 w423]
          frame -2147220623, -2147220621, -2147220364, 56, 63 {
            n146 = One Button Dialog(message="Problem communicating with remote device.  Make sure a valid device is selected and that the IP address is correct.") -> ()  [unwired: 1 in, 1 out]
          }
          frame 1003 {
            n147 = One Button Dialog(message="Dev Error: The Ui.vi for the selected class is broken") -> ()  [unwired: 1 in, 1 out]
          }
          frame 15550 {
            n148 = One Button Dialog(message="The cRIO does not yet have a configuration to download. Create or open a configuration and download it to the cRIO") -> ()  [unwired: 1 in, 1 out]
          }
          frame 537549 {
            n149 = One Button Dialog(message="Invalid configuration file.") -> ()  [unwired: 1 in, 1 out]
            n150 = call <vilib>:"Send Local Message.vi"("message queue in"=w417, "message name"="Exit", "error in"=w416) -> ()  [unwired: 10 in, 3 out]
          }
          frame 538500 {
            n151 = Unbundle By Name(w422) -> ("source"=w421:string)
            n152 = Concatenate Strings("One or more plugin modules were not found. Make sure all plugin modules required to load this configuration have been included in the editor search paths found in 'Tools->Edit Plugin Search Paths'.\n\nOriginal error text:\n " ("message"), w421) -> (w419:string)
            n153 = One Button Dialog(message=w419) -> ()  [unwired: 1 in, 1 out]
          }
          frame Default {
            n154 = call <vilib>:"Simple Error Handler.vi"("error in (no error)"=w423) -> ()  [unwired: 1 in, 8 out]
          }
        }
      }
      frame "Exit" {
        # "Save current path to INI so it will reopen when the editor is launched again"
        # "Stop the VI                                                                             >> Perform any cleanup tasks in this message case. >> Clear display before closing."
        n155 = Unbundle By Name(w429) -> ("current path"=w428:path)
        n156 = call <vilib>:"Destroy Message Queue.vi"("message queue in"=w437, "error in"=w438) -> ("error out"=w433:errorcluster)  [unwired: 11 in, 2 out]
        n157 = control-ref of="Exit"() -> (w435:refnum<vi>)
        n158 = call "Write CurrentPCFG.vi"("File Path"=w428) -> ("Error Out"=w427:errorcluster)  [unwired: 10 in]
        n159 = call "Close DCAF INI.vi"("Error In"=w427) -> ("Error Out"=w426:errorcluster)  [unwired: 10 in]
        n160 = property class="Bool (strict)"(reference=w435, error in=w433, "Val(Sgnl)"=FALSE ("Exit")) -> (error out=w432:errorcluster)  [unwired: 1 out]
        n161 = call <vilib>:"Clear Errors.vi"("error in (no error)"=w426) -> ("error out"=w424:errorcluster)  [unwired: 5 in, 1 out]
        n162 = Merge Errors(w424, w432) -> (w425:errorcluster)
        n163 = call "Remove UI without races.vi"("error in"=w425, "state in"=w429) -> ("error out"=w431:errorcluster, "state out"=w430:T2)  [unwired: 8 in]
        n164 = disable-structure shown="RUN_TIME_ENGINE==True" {
          disable-tunnel: [w439 w440] -> w436
          disable-tunnel: w431 -> [w439 w440]
          frame condition #0 (active) {
          }
          frame condition #1 {
            n165 = Quit LabVIEW() -> ()  [unwired: 1 in]
          }
        }
      }
      frame "------------Menu Operations--------------" {
        # "Dummy case to add a seperation in the Case Structure menu"
      }
      frame "Close?", "DeployTool?", "New?", "Open?" {
        # "Already decided whether to save."
        n166 = Unbundle By Name(w454) -> ("unsaved changes"=w449:bool)
        n167 = case shown="True" w449 {
          tunnel: [TRUE ("SaveFlag") w475] -> w446
          tunnel: w454 -> [w467 w474]
          tunnel: [w467 w473] -> w445
          tunnel: w453 -> [w466 w472]
          tunnel: [w466 w471] -> w450
          tunnel: w448 -> [_ w470]
          tunnel: w443 -> [_ w469]
          frame False {
            # "If there is nothing to save Go do Action"
          }
          frame True {
            n168 = case shown="\"DeployTool?\"" w469 {
              tunnel: [w481 w483] -> w475
              tunnel: w474 -> [w480 w487]
              tunnel: [w479 w482] -> w473
              tunnel: w472 -> [w478 w486]
              tunnel: [w477 w484] -> w471
              tunnel: w470 -> [w476 w485]
              frame Default {
                n169 = call "dialog save dirty dot.vi"("error in"=w478, "View"=w476, "state in"=w480) -> ("error out"=w477:errorcluster, "new"=w481:bool, "state out"=w479:T2)  [unwired: 6 in]
              }
              frame "DeployTool?" {
                n170 = call "dialog save before deploy.vi"("error in"=w486, "View"=w485, "state in"=w487) -> ("error out"=w484:errorcluster, "Continue?"=w483:bool, "state out"=w482:T2)  [unwired: 6 in]
              }
            }
          }
        }
        n171 = Search and Replace String(input string=w443, search string="?", replace string="") -> (result string=w447:string)  [unwired: 5 in, 3 out]
        n172 = case shown="True" w446 {
          tunnel: w450 -> [w458 w465]
          tunnel: [w458 w461] -> w456
          tunnel: w455 -> [_ w464]
          tunnel: w447 -> [_ w463]
          tunnel: w445 -> [w457 w460]
          tunnel: [w457 w459] -> w444
          frame False {
          }
          frame True {
            n173 = call <vilib>:"Send Local Message.vi"("message queue in"=w464, "message name"=w463, "error in"=w465) -> ("error out"=w462:errorcluster)  [unwired: 10 in, 2 out]
            n174 = call "Remove UI without races.vi"("error in"=w462, "state in"=w460) -> ("error out"=w461:errorcluster, "state out"=w459:T2)  [unwired: 8 in]
          }
        }
      }
      frame "New" {
        n175 = Unbundle By Name(w499) -> ("glyph manager"=w498:T9)
        n176 = call "create default cache.vi"() -> ("cache"=w506:T22)  [unwired: 11 in]
        n177 = Unbundle By Name(w506) -> ("configuration.Search Paths"=w505:path[])
        n178 = call-dynamic "AddGlyphtoGManager.vi"("error in"=w500, "glyph manager"=w498, "NISE_CEF_serializable node in"=refnum<class "Systems.lvclass"> refnum ("Systems.lvclass")) -> ("error out"=w501:errorcluster, "glyph manager out"=w497:T9, "NISE_CEF_serializable node out"=w502:refnum<class "Systems.lvclass">)  [unwired: 6 in]
        n179 = call-dynamic "Initialize.vi"("error in"=w501, "node in"=w502) -> ("error out"=w509:errorcluster, "data value reference"=w491:T15)  [unwired: 7 in, 1 out]
        n180 = To More Specific Class(target class=refnum<data-value> refnum, reference=w491, error in=w509) -> (specific class reference=w488:refnum<data-value>, error out=w492:errorcluster)
        n181 = Delete From Array(array=w505) -> (deleted portion=w504:path)  [unwired: 2 in, 1 out]
        n182 = call-dynamic "Initialize.vi"("error in"=w492, "path"=w504, "repository in"=refnum<class "SystemConfigRepo.lvclass"> refnum ("SystemConfigRepo.lvclass")) -> ("error out"=w495:errorcluster, "repository out"=w496:refnum<class "SystemConfigRepo.lvclass">)  [unwired: 7 in]
        n183 = Current VI's Menubar() -> (w493:refnum<k9>)
        n184 = call-dynamic "GenerateMenu.vi"("error in"=w495, "menu ref in"=w493, "SystemConfigRepo in"=w496) -> ("error out"=w494:errorcluster, "SystemConfigRepo out"=w489:refnum<class "SystemConfigRepo.lvclass">)  [unwired: 6 in, 1 out]
        n185 = Bundle By Name(cluster=w499, "unsaved changes"=FALSE ("SaveFlag"), "current path"=path "", "glyph manager"=w497, "root"=w488, "repository"=w489) -> (w512:T2)
        n186 = call <vilib>:"Send Local Message.vi"("message queue in"=w513, "message name"="PopulateTree", "error in"=w494) -> ("error out"=w514:errorcluster)  [unwired: 10 in, 2 out]
      }
      frame "Open" {
        n187 = call <vilib>:"Set Busy.vi"("error in (no error)"=w520) -> ("error out"=w519:errorcluster)  [unwired: 9 in, 1 out]
        n188 = Empty String/Path?(string/path=w515) -> (empty?=w516:bool)
        n189 = case shown="True" w516 {
          tunnel: w523 -> [w530 w540]
          tunnel: w522 -> [w527 w539]
          tunnel: [w526 w535] -> w521
          tunnel: w519 -> [w529 w534]
          tunnel: [w528 w533] -> w518
          tunnel: w515 -> [w524 _]
          frame False {
            # "\"Open\" Message Contains Path Data"
            n190 = String To Path(string=w524) -> (path=w525:path)
            n191 = call "Open PCFG.vi"("error in (no error)"=w529, "Path to PCFG"=w525, "State Cluster"=w530) -> ("error out"=w531:errorcluster, "State Cluster"=w526:T2)  [unwired: 7 in]
            n192 = call <vilib>:"Send Local Message.vi"("message queue in"=w527, "message name"="PopulateTree", "error in"=w531) -> ("error out"=w528:errorcluster)  [unwired: 10 in, 2 out]
          }
          frame True {
            # "\"Open\" Message Does Not Have Data"
            n193 = call "File Dialog"("pattern (all files)"="*.pcfg") -> ("selected path"=w538:path, "cancelled"=w537:bool)  [unwired: 11 in, 2 out]
            n194 = case shown="False" w537 {
              tunnel: w540 -> [w545 w550]
              tunnel: [w544 w550] -> w535
              tunnel: w534 -> [w542 w549]
              tunnel: w539 -> [w548 _]
              tunnel: [w547 w549] -> w533
              tunnel: w538 -> [w541 _]
              frame False {
                # "User Selected .pcfg to Load"
                n195 = call "Open PCFG.vi"("error in (no error)"=w542, "Path to PCFG"=w541, "State Cluster"=w545) -> ("error out"=w543:errorcluster, "State Cluster"=w544:T2)  [unwired: 7 in]
                n196 = call <vilib>:"Send Local Message.vi"("message queue in"=w548, "message name"="PopulateTree", "error in"=w543) -> ("error out"=w547:errorcluster)  [unwired: 10 in, 2 out]
              }
              frame True {
                # "User Cancelled Dialog"
              }
            }
          }
        }
        n197 = call <vilib>:"Unset Busy.vi"("error in (no error)"=w518) -> ("error out"=w517:errorcluster)  [unwired: 10 in]
      }
      frame "Load Binary" {
        n198 = call <vilib>:"Set Busy.vi"("error in (no error)"=w554) -> ("error out"=w553:errorcluster)  [unwired: 9 in, 1 out]
        n199 = call "File Dialog2"("pattern (all files)"="*.pbin") -> ("selected path"=w558:path, "cancelled"=w557:bool)  [unwired: 11 in, 2 out]
        n200 = case shown="False" w557 {
          tunnel: w560 -> [w568 w586]
          tunnel: [w567 w586] -> w555
          tunnel: w553 -> [w566 w585]
          tunnel: w559 -> [w565 _]
          tunnel: [w564 w585] -> w552
          tunnel: w558 -> [w561 _]
          frame False {
            n201 = in-place {
              in-place-border: w566 -> [w577]
              in-place-border: [w569] -> w562
              in-place-border: w561 -> [w578]
              n202 = in-place-cluster #3(w568) -> ("repository"=w579:refnum<class "SystemConfigRepo.lvclass">)  [unwired: 2 out]
              n203 = call <vilib>:"read full file.vi"("error in"=w577, "file path"=w578) -> ("error out"=w576:errorcluster, "data"=w575:string)  [unwired: 8 in]
              n204 = call <vilib>:"unflatten memory.vi"("error in"=w576, "binary repo"=w575, "NISE_CEF_HierarchyRepo in"=w579) -> ("error out"=w580:errorcluster, "NISE_CEF_HierarchyRepo out"=w581:refnum<class "SystemConfigRepo.lvclass">)  [unwired: 7 in]
              n205 = call-dynamic "WriteTree.vi"("error in"=w580, "repository in"=w581) -> ("error out"=w571:errorcluster, "root"=w574:T15, "repository out"=w583:refnum<class "NISE_CEF_Repository.lvclass">)  [unwired: 7 in]
              n206 = To More Specific Class(target class=w579, reference=w583, error in=w571) -> (specific class reference=w582:refnum<class "SystemConfigRepo.lvclass">, error out=w570:errorcluster)
              n207 = To More Specific Class(target class=refnum<data-value> refnum, reference=w574, error in=w570) -> (specific class reference=w573:refnum<data-value>, error out=w569:errorcluster)
              n208 = in-place-cluster #3("unsaved changes"=TRUE ("SaveFlag"), "repository"=w582, "root"=w573) -> (w567:T2)
            }
            n209 = call <vilib>:"Send Local Message.vi"("message queue in"=w565, "message name"="PopulateTree", "error in"=w562) -> ("error out"=w564:errorcluster)  [unwired: 10 in, 2 out]
          }
          frame True {
          }
        }
        n210 = call <vilib>:"Unset Busy.vi"("error in (no error)"=w552) -> ("error out"=w551:errorcluster)  [unwired: 10 in]
      }
      frame "Save", "SaveAs" {
        n211 = call "Remove UI without races.vi"("error in"=w597, "state in"=w595) -> ("error out"=w593:errorcluster, "state out"=w594:T2)  [unwired: 8 in]
        n212 = call <vilib>:"Set Busy.vi"("error in (no error)"=w593) -> ("error out"=w592:errorcluster)  [unwired: 9 in, 1 out]
        n213 = Equal?(x="SaveAs", y=w599) -> (x = y?=w589:bool)
        n214 = local read "View"() -> (w587:string)
        n215 = call "save operation.vi"("force save as"=w589, "error in"=w592, "state cluster"=w594) -> ("error out"=w598:errorcluster, "state out"=w602:T2)  [unwired: 7 in]
        n216 = property on="View" class="Tree (strict)"(error in=w598, "Val(Sgnl)"=w587) -> (error out=w591:errorcluster)  [unwired: 1 in, 1 out]
        n217 = call <vilib>:"Unset Busy.vi"("error in (no error)"=w591) -> ("error out"=w590:errorcluster)  [unwired: 10 in]
        n218 = call <vilib>:"Send Local Message.vi"("message queue in"=w596, "message name"="PopulateTree", "error in"=w590) -> ("error out"=w601:errorcluster)  [unwired: 10 in, 2 out]
      }
      frame "Save Binary" {
        n219 = call "Remove UI without races.vi"("error in"=w609, "state in"=w608) -> ("error out"=w606:errorcluster, "state out"=w607:T2)  [unwired: 8 in]
        n220 = call <vilib>:"Set Busy.vi"("error in (no error)"=w606) -> ("error out"=w611:errorcluster)  [unwired: 9 in, 1 out]
        n221 = local read "View"() -> (w603:string)
        n222 = call "save operation binary.vi"("error in"=w611, "state cluster"=w607) -> ("error out"=w610:errorcluster, "state out"=w615:T2)  [unwired: 8 in]
        n223 = property on="View" class="Tree (strict)"(error in=w610, "Val(Sgnl)"=w603) -> (error out=w604:errorcluster)  [unwired: 1 in, 1 out]
        n224 = call <vilib>:"Unset Busy.vi"("error in (no error)"=w604) -> ("error out"=w605:errorcluster)  [unwired: 10 in]
        n225 = call <vilib>:"Send Local Message.vi"("message queue in"=w613, "message name"="PopulateTree", "error in"=w605) -> ("error out"=w614:errorcluster)  [unwired: 10 in, 2 out]
      }
      frame "Custom View" {
        n226 = in-place {
          in-place-border: w623 -> [w639]
          in-place-border: [w631] -> w616
          in-place-border: w618 -> [w632]
          n227 = in-place-cluster #4(w620) -> ("repository"=w629:refnum<class "SystemConfigRepo.lvclass">, "root"=w637:refnum<data-value>)
          n228 = call-dynamic "ReadTree.vi"("error in"=w639, "root"=w637, "repository in"=w629) -> ("error out"=w636:errorcluster, "repository out"=w634:refnum<class "NISE_CEF_Repository.lvclass">)  [unwired: 7 in]
          n229 = call-dynamic "CustomView.vi"("error in"=w636, "view name"=w632, "repository in"=w634) -> ("error out"=w635:errorcluster, "repository out"=w633:refnum<class "NISE_CEF_Repository.lvclass">)  [unwired: 7 in]
          n230 = call-dynamic "WriteTree.vi"("error in"=w635, "repository in"=w633) -> ("error out"=w638:errorcluster, "root"=w626:T15, "repository out"=w630:refnum<class "NISE_CEF_Repository.lvclass">)  [unwired: 7 in]
          n231 = To More Specific Class(target class=refnum<data-value> refnum, reference=w626, error in=w638) -> (specific class reference=w624:refnum<data-value>, error out=w627:errorcluster)
          n232 = To More Specific Class(target class=w629, reference=w630, error in=w627) -> (specific class reference=w628:refnum<class "SystemConfigRepo.lvclass">, error out=w631:errorcluster)
          n233 = in-place-cluster #4("repository"=w628, "root"=w624) -> (w619:T2)
        }
        n234 = call <vilib>:"Send Local Message.vi"("message queue in"=w621, "message name"="PopulateTree", "error in"=w616) -> ("error out"=w622:errorcluster)  [unwired: 10 in, 2 out]
      }
      frame "DeployTool" {
        n235 = Unbundle By Name(w644) -> ("current path"=w640:path, "root"=w641:refnum<data-value>)
        n236 = call "deployment tool.vi"("current pcfg path"=w640, "error in"=w643, "root"=w641) -> ("error out"=w642:errorcluster)  [unwired: 8 in]
      }
      frame "Edit Plugin Search Paths" {
        n237 = Unbundle By Name(w662) -> ("current path"=w654:path, "repository"=w655:refnum<class "SystemConfigRepo.lvclass">, "classes cache"=w660:path)
        n238 = call "load cache.vi"("error in"=w661, "cache path"=w660) -> ("error out"=w659:errorcluster, "cache"=w657:T22)  [unwired: 8 in]
        n239 = case shown="Error" w659 {
          selector: w659 -> [w672 _]
          tunnel: [w673 w674] -> w658
          tunnel: w657 -> [w673 _]
          tunnel: [w672 _] -> w656
          frame No Error {
          }
          frame Error {
            n240 = call "create default cache.vi"() -> ("cache"=w674:T22)  [unwired: 11 in]
          }
        }
        n241 = Path To String(path=w654) -> (string=w647:string)
        n242 = call "Check for Missing Modules.vi"("SystemConfigRepo in"=w655) -> ("Missing Module?"=w653:bool)  [unwired: 9 in, 1 out]
        n243 = Unbundle By Name(w658) -> ("configuration.Search Paths"=w665:path[])
        n244 = call "dialog edit search paths.vi"("error in"=w656, "Plugin Search Paths"=w665) -> ("error out"=w663:errorcluster, "Cancelled?"=w651:bool, "Plugin Search Paths"=w664:path[])  [unwired: 7 in]
        n245 = case shown="False" w651 {
          tunnel: w658 -> [w685 _]
          tunnel: w664 -> [w684 _]
          tunnel: w663 -> [w678 w687]
          tunnel: w646 -> [w681 w686]
          tunnel: [w680 w687] -> w650
          tunnel: w660 -> [w676 _]
          tunnel: [w675 w686] -> w645
          frame False {
            n246 = Bundle By Name(cluster=w685, "configuration.Search Paths"=w684) -> (w677:T22)
            n247 = call "save cache.vi"("error in"=w678, "cache"=w677, "path"=w676) -> ("error out"=w679:errorcluster)  [unwired: 8 in]
            n248 = call <vilib>:"Send Local Message.vi"("message queue in"=w681, "message name"="FindPluginNodes", "message value"="Refresh", "error in"=w679) -> ("message queue out"=w675:T11, "error out"=w680:errorcluster)  [unwired: 9 in, 1 out]
          }
          frame True {
          }
        }
        n249 = Not(x=w651) -> (.not. x?=w652:bool)
        n250 = And(x=w653, y=w652) -> (x .and. y?=w648:bool)
        n251 = case shown="True" w648 {
          tunnel: w650 -> [w666 w671]
          tunnel: [w666 w670] -> w649
          tunnel: w647 -> [_ w669]
          tunnel: w645 -> [_ w667]
          frame False {
          }
          frame True {
            n252 = call <vilib>:"Send Local Message.vi"("message queue in"=w667, "message name"="Open" ("message value"), "message value"=w669, "error in"=w671) -> ("error out"=w670:errorcluster)  [unwired: 9 in, 2 out]
          }
        }
      }
      frame "FindPluginNodes" {
        n253 = call <vilib>:"Set Busy.vi"("error in (no error)"=w691) -> ("error out"=w690:errorcluster)  [unwired: 9 in, 1 out]
        n254 = Unbundle By Name(w717) -> ("classes cache"=w710:path)
        n255 = call <vilib>:"Launch Progress Bar.vi"("error in (no error)"=w690) -> ("error out"=w695:errorcluster, "Exists?"=w692:bool)  [unwired: 9 in]
        n256 = case shown="False" w692 {
          tunnel: w695 -> [w720 w723]
          tunnel: [w719 w723] -> w694
          tunnel: [u8 0 ("Value") u8 45 ("Value")] -> w693
          frame False {
            n257 = call <vilib>:"Set Title Text.vi"("error in (no error)"=w720, "Installer Title"="Refreshing Plugins") -> ("error out"=w719:errorcluster)  [unwired: 9 in]
          }
          frame True {
          }
        }
        n258 = To Lower Case(string="Refresh" ("x")) -> (all lower case string=w708:string)
        n259 = To Lower Case(string=w716) -> (all lower case string=w707:string)
        n260 = call "load cache.vi"("error in"=w690, "cache path"=w710) -> ("error out"=w714:errorcluster, "cache"=w713:T22)  [unwired: 8 in]
        n261 = Equal?(x=w708, y=w707) -> (x = y?=w711:bool)
        n262 = case shown="Error" w714 {
          selector: w714 -> [w729 _]
          tunnel: [w727 w730] -> w712
          tunnel: w713 -> [w728 _]
          tunnel: [w729 _] -> w701
          frame No Error {
            n263 = call "remove missing files.vi"("cache in"=w728) -> ("cache out"=w727:T22)  [unwired: 10 in]
          }
          frame Error {
            n264 = call "create default cache.vi"() -> ("cache"=w730:T22)  [unwired: 11 in]
          }
        }
        n265 = call <vilib>:"Update Progress Bar.vi"("Action"=Update_Bar_Actions."Set to Value", "error in (no error)"=w694, "Value"=w693) -> ("error out"=w706:errorcluster)  [unwired: 8 in]
        n266 = call <vilib>:"Set Action Text.vi"("error in (no error)"=w706, "Action Text"="Loading Classes...") -> ("error out"=w705:errorcluster)  [unwired: 9 in]
        n267 = call <vilib>:"Clear Errors.vi"("error in (no error)"=w705) -> ("error out"=w702:errorcluster)  [unwired: 5 in, 1 out]
        n268 = Merge Errors(w701, w702) -> (w700:errorcluster)
        n269 = call "identify new classes.vi"("existing progress bar?"=w692, "error in"=w700, "force scan"=w711, "cache in"=w712) -> ("error out"=w698:errorcluster, "cache out"=w709:T22)  [unwired: 6 in]
        n270 = call <vilib>:"Set Action Text.vi"("error in (no error)"=w698, "Action Text"="Saving Cache...") -> ("error out"=w697:errorcluster)  [unwired: 9 in]
        n271 = call "save cache.vi"("error in"=w697, "cache"=w709, "path"=w710) -> ("error out"=w689:errorcluster)  [unwired: 8 in]
        n272 = call <vilib>:"Unset Busy.vi"("error in (no error)"=w689) -> ("error out"=w688:errorcluster)  [unwired: 10 in]
        n273 = case shown="False" w692 {
          tunnel: w688 -> [w725 w726]
          tunnel: [w724 w726] -> w696
          frame False {
            n274 = call <vilib>:"Close Progress Bar.vi"("error in (no error)"=w725) -> ("error out"=w724:errorcluster)  [unwired: 9 in, 1 out]
          }
          frame True {
          }
        }
      }
      frame "Test" {
        n275 = in-place {
          in-place-border: w737 -> [w752]
          in-place-border: [w748] -> w731
          n276 = in-place-cluster #5(w734) -> ("repository"=w743:refnum<class "SystemConfigRepo.lvclass">, "root"=w750:refnum<data-value>)
          n277 = call-dynamic "ReadTree.vi"("error in"=w752, "root"=w750, "repository in"=w743) -> ("error out"=w749:errorcluster, "repository out"=w745:refnum<class "NISE_CEF_Repository.lvclass">)  [unwired: 7 in]
          n278 = To More Specific Class(target class=w743, reference=w745, error in=w749) -> (specific class reference=w744:refnum<class "SystemConfigRepo.lvclass">, error out=w746:errorcluster)
          n279 = call-dynamic "WriteTree.vi"("error in"=w746, "repository in"=w744) -> ("error out"=w751:errorcluster, "root"=w740:T15, "repository out"=w747:refnum<class "NISE_CEF_Repository.lvclass">)  [unwired: 7 in]
          n280 = To More Specific Class(target class=refnum<data-value> refnum, reference=w740, error in=w751) -> (specific class reference=w739:refnum<data-value>, error out=w741:errorcluster)
          n281 = To More Specific Class(target class=w743, reference=w747, error in=w741) -> (specific class reference=w742:refnum<class "SystemConfigRepo.lvclass">, error out=w748:errorcluster)
          n282 = in-place-cluster #5("repository"=w742, "root"=w739) -> (w733:T2)
        }
        n283 = call <vilib>:"Send Local Message.vi"("message queue in"=w735, "message name"="PopulateTree", "error in"=w731) -> ("error out"=w736:errorcluster)  [unwired: 10 in, 2 out]
      }
      frame "HandleMenu" {
        n284 = Unflatten From String(type=T12 {"node id"="", "RightClickPath"=""} ("input cluster"), binary string=w774, error in (no error)=w775) -> (value=w772:T12, error out=w753:errorcluster)  [unwired: 2 in, 1 out]
        n285 = Unbundle By Name(w772) -> ("RightClickPath"=w768:string, "node id"=w771:string)
        n286 = call <vilib>:"IDtoNode.vi"("error in"=w753, "ID"=w771) -> ("error out"=w770:errorcluster, "node ref"=w757:T15)  [unwired: 7 in, 1 out]
        n287 = Unbundle By Name(w762) -> ("unsaved changes"=w760:bool, "standard events.node change"=w755:T5)
        n288 = in-place {
          in-place-border: w770 -> [w802]
          in-place-border: [w799] -> w763
          in-place-border: [w798] -> w769
          in-place-border: w768 -> [w797]
          in-place-border: [w797] -> w767
          in-place-border: w766 -> [w796]
          in-place-border: w765 -> [w795]
          in-place-border: [w792] -> w759
          in-place-border: [w791] -> w756
          n289 = in-place-dvr #6(w757) -> (w793:refnum<class "NISE_CEF_Node.lvclass">, w801:errorcluster)
          n290 = Merge Errors(w801, w802) -> (w800:errorcluster)
          n291 = call-dynamic "MenuHandler.vi"("tree control"=w795, "main message queue"=w796, "error in"=w800, "menu string"=w797, "NISE_CEF_Node in"=w793) -> ("error out"=w799:errorcluster, "refresh tree?"=w791:bool, "Unhandled"=w798:bool, "NISE_CEF_Node out"=w794:refnum<class "NISE_CEF_Node.lvclass">)  [unwired: 3 in]
          n292 = Not Equal?(x=w793, y=w794) -> (x != y?=w792:bool)
          n293 = in-place-dvr #6(w794) -> (w754:T15)  [unwired: 1 out]
        }
        n294 = Or(x=w760, y=w759) -> (x .or. y?=w758:bool)
        n295 = Bundle By Name(cluster=w762, "unsaved changes"=w758) -> (w761:T2)
        n296 = case shown="True" w769 {
          tunnel: w767 -> [_ w786]
          tunnel: [w779 w788] -> w764
          tunnel: w763 -> [w778 w787]
          tunnel: w756 -> [w780 _]
          tunnel: w755 -> [w777 _]
          tunnel: w754 -> [w776 _]
          frame False {
            n297 = case shown="True" w780 {
              tunnel: [w781 w784] -> w779
              tunnel: w778 -> [w781 w785]
              tunnel: w777 -> [_ w783]
              tunnel: w776 -> [_ w782]
              frame False {
              }
              frame True {
                n298 = Generate User Event(user event=w783, event data cluster=w782, error in=w785) -> (error out=w784:errorcluster)  [unwired: 1 in, 1 out]
              }
            }
          }
          frame True {
            n299 = call <vilib>:"NISE_error generator.vi"("error in"=w787, "source"="configuration tool main.vi", "append error message"=w786, "error code (0)"=538506) -> ("error out"=w788:errorcluster)  [unwired: 5 in]
          }
        }
      }
      frame "EditorMenu" {
        n300 = Unbundle By Name(w813) -> ("repository"=w810:refnum<class "SystemConfigRepo.lvclass">)
        n301 = Unflatten From String(type=cluster{"ItemTag":string, string} {"ItemTag"="", ""} ("anything"), binary string=w816, error in (no error)=w817) -> (value=w814:cluster{"ItemTag":string, string}, error out=w811:errorcluster)  [unwired: 2 in, 1 out]
        n302 = Unbundle(w814) -> ("ItemTag"=w808:string, w803:string)
        n303 = call-dynamic "HandleMenu.vi"("message queue"=w809, "error in"=w811, "Item Path"=w803, "ItemTag"=w808, "NISE_CEF_Repository in"=w810) -> ("error out"=w805:errorcluster, "handled?"=w806:bool, "NISE_CEF_Repository out"=w807:refnum<class "SystemConfigRepo.lvclass">)  [unwired: 4 in]
        n304 = case shown="False" w806 {
          tunnel: w805 -> [w819 w823]
          tunnel: [w820 w823] -> w804
          tunnel: w803 -> [w818 _]
          frame False {
            n305 = call <vilib>:"NISE_error generator.vi"("error in"=w819, "source"="configuration tool main.vi", "append error message"=w818, "error code (0)"=538506) -> ("error out"=w820:errorcluster)  [unwired: 5 in]
          }
          frame True {
          }
        }
        n306 = Bundle By Name(cluster=w813, "repository"=w807) -> (w812:T2)
      }
      frame "Script Include VI" {
        n307 = call "call include vi script.vi"("error in"=w825, "state cluster"=w826) -> ("error out"=w824:errorcluster)  [unwired: 9 in]
      }
      frame "-------TreeControl Operations-----------" {
        # "Dummy case to add a seperation in the Case Structure menu"
      }
      frame "AddNode" {
        n308 = call <vilib>:"Set Busy.vi"("error in (no error)"=w838) -> ("error out"=w837:errorcluster)  [unwired: 9 in, 1 out]
        n309 = Unflatten From String(type=T13 {"node type"="", "to add to"=""} ("input cluster"), binary string=w860) -> (value=w856:T13)  [unwired: 3 in, 2 out]
        n310 = Unbundle By Name(w856) -> ("to add to"=w854:string, "node type"=w833:string)
        n311 = Match Pattern(string=w833, regular expression=":") -> (after substring=w836:string, offset past match=w835:i32)  [unwired: 1 in, 2 out]
        n312 = Unbundle By Name(w831) -> ("glyph manager"=w829:T9, "repository"=w830:refnum<class "SystemConfigRepo.lvclass">)
        n313 = case shown="-1" w835 {
          tunnel: w833 -> [_ w862]
          tunnel: [w861 w862] -> w832
          tunnel: w836 -> [w861 _]
          frame 0, Default {
          }
          frame -1 {
          }
        }
        n314 = call-dynamic "GetClassPath.vi"("error in"=w837, "class name"=w832, "Repository in"=w830) -> ("error out"=w850:errorcluster, "class path"=w851:path)  [unwired: 6 in, 1 out]
        n315 = call <vilib>:"Get LV Class Default Value.vi"("error in (no error)"=w850, "class path"=w851) -> ("error out"=w858:errorcluster, "object"=w859:refnum<class>)  [unwired: 8 in]
        n316 = To More Specific Class(target class=refnum<class "NISE_CEF_Node.lvclass"> refnum ("NISE_CEF_Node.lvclass"), reference=w859, error in=w858) -> (specific class reference=w844:refnum<class "NISE_CEF_Node.lvclass">, error out=w845:errorcluster)
        n317 = call-dynamic "AddGlyphtoGManager.vi"("error in"=w845, "glyph manager"=w829, "NISE_CEF_Node in"=w844) -> ("error out"=w842:errorcluster, "glyph manager out"=w841:T9, "NISE_CEF_Node out"=w843:refnum<class "NISE_CEF_Node.lvclass">)  [unwired: 6 in]
        n318 = call <vilib>:"AddNode.vi"("error in"=w842, "node in"=w843, "parent node ID"=w854) -> ("error out"=w853:errorcluster, "summary"=w852:T28[])  [unwired: 7 in]
        n319 = call <vilib>:"PopulateTreeSumaryWithGlyphManager.vi"("error in"=w853, "glyph manager"=w841, "summary"=w852, "tree ref in"=w849) -> ("error out"=w840:errorcluster, "glyph manager out"=w846:T9)  [unwired: 6 in]
        n320 = call <vilib>:"Unset Busy.vi"("error in (no error)"=w840) -> ("error out"=w839:errorcluster)  [unwired: 10 in]
        n321 = Bundle By Name(cluster=w831, "unsaved changes"=TRUE, "glyph manager"=w846) -> (w848:T2)
      }
      frame "Duplicate" {
        n322 = call <vilib>:"IDtoNode.vi"("error in"=w873, "ID"=w874) -> ("error out"=w871:errorcluster, "invalid Id"=w870:bool, "node ref"=w872:T15)  [unwired: 7 in]
        n323 = Unbundle By Name(w866) -> ("glyph manager"=w865:T9)
        n324 = case shown="False" w870 {
          tunnel: [w876 w890] -> w863
          tunnel: w872 -> [w877 _]
          tunnel: w871 -> [w888 w890]
          tunnel: w869 -> [w884 _]
          tunnel: w865 -> [w882 w889]
          tunnel: [w883 w889] -> w864
          frame False {
            n325 = call <vilib>:"DuplicateNode.vi"("same parent?"=TRUE ("s"), "error in"=w888, "node ref in"=w877) -> ("error out"=w878:errorcluster, "new node ref"=w880:T15)  [unwired: 7 in]
            n326 = call "clean duplicated node mappings.vi"("error in (no error)"=w878, "Old Node"=w877, "New Node"=w880) -> ("error out"=w879:errorcluster, "New Node"=w875:T15)  [unwired: 6 in, 1 out]
            n327 = call <vilib>:"SummaryWithGlyphManager.vi"("error in"=w879, "glyph manager"=w882, "node self ref"=w875) -> ("error out"=w886:errorcluster, "glyph manager out"=w881:T9, "summary"=w885:T28[])  [unwired: 6 in]
            n328 = call <vilib>:"PopulateTreeSumaryWithGlyphManager.vi"("error in"=w886, "glyph manager"=w881, "summary"=w885, "tree ref in"=w884) -> ("error out"=w876:errorcluster, "glyph manager out"=w883:T9)  [unwired: 6 in]
          }
          frame True {
          }
        }
        n329 = Bundle By Name(cluster=w866, "unsaved changes"=TRUE, "glyph manager"=w864) -> (w868:T2)
      }
      frame "RefreshNode" {
        # "Refreshes the node in the Tree               Sets the save flag to true                       This case can be called from the UIs of the nodes"
        n330 = Unbundle By Name(w894) -> ("glyph manager"=w893:T9)
        n331 = call <vilib>:"IDtoNode.vi"("error in"=w899, "ID"=w898) -> ("error out"=w897:errorcluster, "invalid Id"=w896:bool, "node ref"=w891:T15)  [unwired: 7 in]
        n332 = case shown="False" w896 {
          tunnel: [w904 w913] -> w901
          tunnel: w897 -> [w910 w913]
          tunnel: w891 -> [w903 _]
          tunnel: w895 -> [w909 _]
          tunnel: w893 -> [w906 w912]
          tunnel: [w908 w912] -> w892
          frame False {
            n333 = call <vilib>:"SummaryWithGlyphManager.vi"("error in"=w910, "glyph manager"=w906, "node self ref"=w903) -> ("error out"=w911:errorcluster, "glyph manager out"=w907:T9, "summary"=w902:T28[])  [unwired: 6 in]
            n334 = call <vilib>:"RefreshSubTreeWithGlyphManager.vi"("error in"=w911, "glyph manager"=w907, "node information"=w902, "tree ref in"=w909) -> ("error out"=w905:errorcluster, "glyph manager out"=w908:T9)  [unwired: 5 in, 1 out]
            n335 = call "Refresh All Nodes.vi"("error in (no error)"=w905, "summary"=w902) -> ("error out"=w904:errorcluster)  [unwired: 9 in]
          }
          frame True {
          }
        }
        n336 = Bundle By Name(cluster=w894, "glyph manager"=w892) -> (w900:T2)
      }
      frame "SetDirtyDot" {
        n337 = Bundle By Name(cluster=w917, "unsaved changes"=TRUE ("SaveFlag")) -> (w916:T2)
      }
      frame "RemoveNode" {
        n338 = call <vilib>:"IDtoNode.vi"("error in"=w928, "ID"=w929) -> ("error out"=w926:errorcluster, "invalid Id"=w924:bool, "node ref"=w925:T15)  [unwired: 7 in]
        n339 = case shown="False" w924 {
          tunnel: w926 -> [w938 w950]
          tunnel: w925 -> [w936 _]
          tunnel: [w940 w950] -> w927
          tunnel: w923 -> [w939 _]
          tunnel: w922 -> [w935 _]
          tunnel: w919 -> [w931 w949]
          tunnel: [w930 w949] -> w918
          frame False {
            n340 = call "check if subpanel should be closed.vi"("error in"=w938, "SubPanel in"=w935, "node in"=w936) -> ("error out"=w934:errorcluster, "needs closing"=w932:bool, "node out"=w937:T15)  [unwired: 6 in]
            n341 = case shown="False" w932 {
              tunnel: w935 -> [_ _]
              tunnel: w934 -> [w944 w948]
              tunnel: [w944 w947] -> w933
              tunnel: w931 -> [w943 w946]
              tunnel: [w943 w945] -> w930
              frame False {
              }
              frame True {
                n342 = call "Remove UI without races.vi"("error in"=w948, "state in"=w946) -> ("error out"=w947:errorcluster, "state out"=w945:T2)  [unwired: 8 in]
              }
            }
            n343 = call <vilib>:"RemoveNode.vi"("error in"=w933, "node"=w937) -> ("error out"=w941:errorcluster, "node ID"=w942:string)  [unwired: 8 in]
            n344 = call <vilib>:"ClearTreeNode.vi"("error in"=w941, "tag"=w942, "tree reference"=w939) -> ("error out"=w940:errorcluster)  [unwired: 8 in]
          }
          frame True {
          }
        }
        n345 = Bundle By Name(cluster=w918, "unsaved changes"=TRUE) -> (w921:T2)
      }
      frame "PopulateTree" {
        w954 = "DCAF Editor" ("f")
        n346 = Unbundle By Name(w976) -> ("current path"=w960:path, "root"=w973:refnum<data-value>, "glyph manager"=w957:T9)
        n347 = call <vilib>:"SummaryWithGlyphManager.vi"("error in"=w971, "glyph manager"=w957, "depth"=0 ("Depth"), "node self ref"=w973) -> ("error out"=w974:errorcluster, "glyph manager out"=w962:T9, "summary"=w975:T28[])  [unwired: 5 in]
        n348 = call <vilib>:"Check if File or Folder Exists.vi"("path"=w960) -> ("file or folder exists?"=w965:bool, "dup path"=w967:path)  [unwired: 8 in, 1 out]
        n349 = Empty String/Path?(string/path=w960) -> (empty?=w961:bool)
        n350 = Equal?(x=w960, y=path "") -> (x = y?=w958:bool)
        n351 = call <vilib>:"RefreshEntireTreeWithGlyphManager.vi"("calling VI in"=w956, "error in"=w974, "glyph manager"=w962, "array"=w975, "tree ref in"=w970) -> ("error out"=w969:errorcluster, "glyph manager out"=w963:T9)  [unwired: 5 in]
        n352 = Compound Arithmetic op=AND(w965, invert w961, invert w958) -> (w951:bool)
        n353 = Strip Path(path=w967) -> (name=w953:string)  [unwired: 1 out]
        n354 = Format Into String(format string="%s - %s", w953, w954) -> (resulting string=w952:string)  [unwired: 2 in, 1 out]
        n355 = Select(t=w952, s=w951, f=w954) -> (s? t:f=w966:string)
        n356 = Bundle By Name(cluster=w976, "glyph manager"=w963) -> (w964:T2)
        n357 = property class="VI"(reference=w956, error in=w969, "Front Panel.Title"=w966) -> (error out=w968:errorcluster)  [unwired: 1 out]
      }
      frame "CleansubPanel" {
        n358 = call "Remove UI without races.vi"("error in"=w980, "state in"=w978) -> ("error out"=w979:errorcluster, "state out"=w977:T2)  [unwired: 8 in]
      }
      frame "ActivateNode" {
        n359 = call <vilib>:"Set Busy.vi"("error in (no error)"=w989) -> ("error out"=w984:errorcluster)  [unwired: 9 in, 1 out]
        n360 = call <vilib>:"IDtoNode.vi"("error in"=w984, "ID"=w990) -> ("error out"=w985:errorcluster, "invalid Id"=w987:bool, "node ref"=w986:T15)  [unwired: 7 in]
        n361 = case shown="False" w987 {
          tunnel: w986 -> [w993 _]
          tunnel: [w997 w999] -> w983
          tunnel: w985 -> [w995 w999]
          tunnel: [w994 w998] -> w982
          tunnel: w981 -> [w991 w998]
          frame False {
            n362 = call "Remove UI without races.vi"("error in"=w995, "state in"=w991) -> ("error out"=w996:errorcluster, "state out"=w992:T2)  [unwired: 8 in]
            n363 = call "Load node UI optimized.vi"("error in"=w996, "node"=w993, "state in"=w992) -> ("error out"=w997:errorcluster, "state out"=w994:T2)  [unwired: 7 in]
          }
          frame True {
          }
        }
        n364 = call <vilib>:"Unset Busy.vi"("error in (no error)"=w983) -> ("error out"=w988:errorcluster)  [unwired: 10 in]
      }
      frame "Move" {
        n365 = call "Move Node.vi"("error in (no error)"=w1006, "message value"=w1007) -> ("error out"=w1002:errorcluster)  [unwired: 9 in]
        n366 = Bundle By Name(cluster=w1008, "unsaved changes"=TRUE) -> (w1001:T2)
        n367 = call <vilib>:"Send Local Message.vi"("message queue in"=w1004, "message name"="PopulateTree", "error in"=w1002) -> ("error out"=w1005:errorcluster)  [unwired: 10 in, 2 out]
      }
      frame "RefreshNodeView" {
        # "This user event is used by editor nodes to update their subpanels when data in the tree changes."
        n368 = Unbundle By Name(w1012) -> ("standard events.refresh UI"=w1010:T7)
        n369 = Generate User Event(user event=w1010, event data cluster=TRUE ("event data"), error in=w1013) -> (error out=w1011:errorcluster)  [unwired: 1 in, 1 out]
      }
      frame "NodeDataChange" {
        n370 = call <vilib>:"Send Local Message.vi"("message queue in"=w1017, "message name"="RefreshNode", "message value"=w1016, "error in"=w1019) -> ("error out"=w1018:errorcluster)  [unwired: 9 in, 2 out]
        n371 = Bundle By Name(cluster=w1021, "unsaved changes"=TRUE) -> (w1015:T2)
      }
    }
  }
  n372 = Unregister For Events(event registration refnum=w11) -> ()  [unwired: 1 in, 1 out]
  n373 = call <vilib>:"DestroyStandardEvents.vi"("error in"=w10, "standard events"=w9) -> ()  [unwired: 9 in, 1 out]
